vi "WildBugChilGru.vi"() -> ()   [LabVIEW 2014]
uses:
  <vilib>/Utility/miscctls.llb/LVPointTypeDef.ctl
  <vilib>/Utility/xml.llb/Write to XML File(string).vi
  <vilib>/Platform/browser.llb/Open URL in Default Browser (string).vi
  <vilib>/Instr/_visa.llb/VISA Configure Serial Port (Instr).vi
  <vilib>/Analysis/3filter.llb/IIR Filter (DBL).vi
  <vilib>/gmath/NI_Gmath.lvlib
  <vilib>/Analysis/NI_AALBase.lvlib
  <vilib>/ptbypt/NI_PtbyPt.lvlib
panel:
  in  "Grossbild schließen":bool=TRUE
  out "Fahrzeugdaten_gross":string="Fahrzeugdaten"
  out "(c)_gross":string="\n  (c) WildBugGruChil, germanscooterforum.de"
  out "nM_gross":string="\n    4235 1/min"
  out "M_gross":string="15,4 Nm"
  out "Titel_gross":string="Titel"
  out "PS_gross":string="37,6 PS"
  out "nPS_gross":string="\n  6575 1/min"
  out "Y-Koord. Graph-Reset-Button (782)":i32=782
  out "Höhe Leistungs-Graph (646)":u32=646
  in  "FahrzeugdatenZeichenzahl":u8 max=100
  out "Strecke [m]":dbl
  out "dT":dbl=3003.0
  out "Cyclecounter":dbl=3003.0
  out "Datum+Zeit":string="01.12.2021 09:48"
  out "n(Pmax)":dbl=5307.692307692308
  out "Pmax":dbl=17.77254327549455
  out "Lauf abgebrochen":bool
  out "Auto-Datei":string
  out "Auto-Gespeichert":bool
  in  "Auto-Pfad":path
  in  "Auto-Speichern":bool
  out "n(Rolle) [1/min]":dbl=3003.0
  in  "Fahrzeugdaten":string
  out "Ergebnis":string
  out "Pmax":string
  in  "Drucken":bool
  in  "Speichern":bool
  in  "Start":bool
  in  "Ende":bool
  in  "Spenden":bool
  in  "Registerkarte":T1(tab)=enum."Betriebsmodus & Recalc"
  in  "Zündung [Imp/U]":dbl=1.0 format="%#.2f"
  in  "Übersetzung ermitteln aus":T2(ring)
  in  "Getriebe [1:]":dbl=4.0 min=0.0001
  in  "Reifenumfang [m]":dbl=1.222 min=0.0001
  in  "Dauer [s]":u8=5
  in  "nKuWe/nRolle":dbl=0.8 format="%#.3f"
  in  "Lufttemperatur [°C]":dbl=23.2 format="%#.1g"
  in  "Luftdruck [mbar]":dbl=100.34 min=0.0001
  in  "Messung Klimadaten":bool=TRUE
  in  "Filter Zündsignal":bool
  in  "v vom Gas [km/h]":u16=40
  in  "Gleitender Mittelwert":u8=35
  in  "Differenzenquotient":u8=12
  in  "n vom Gas [1/min]":u16=5000
  in  "Verlustmoment M1 [Nm] bei n1":dbl min=0.0
  in  "Rollendrehzahl n1 [1/min]":u16=1 min=1
  in  "Verlustmoment M0 [Nm] bei n = 0":dbl min=0.0
  in  "Rollengeber [Inkr/U]":u16=20 min=1
  in  "Rollenumfang [m]":dbl=0.5 min=0.0001
  in  "Rollenträgheit [kgm²]":dbl=2.0 min=0.0001
  in  "Rollendrehzahl aufzeichnen":bool
  in  "Überschrift Leistungsdiagramm":string
  in  "Recalc":bool
  in  "Leistung":bool=TRUE caption="Messung Klimadaten"
  in  "AFR, EGT":bool caption="Messung Klimadaten"
  in  "Lambda":bool caption="Messung Klimadaten"
  in  "Grossbild":bool
  out "Datenspeicher":T3={"Fahrzeugdaten"="§$", "Auto-Pfad"="01.12.2021 09:48|", "Rolle [Inkr/U]"=20, "Rollenumfang [m]"=0.5, "Rollenträgheit [kgm²]"=2.0, "Zündung [Imp/U]"=1.0, "Getriebe [1:]"=4.0, "Reifenumfang [m] "=1.222, "Grossanzeige"=0.0, "Gl. Mittelwert"=35, "Differenzenquotient"=12, "AFR,EGT"=0, "dT [s]"=0.02, "Strecke [m]"=405.045585106383, "Lufttemperatur [°C]"=23.2, "Mv: n1 [1/min]"=1.0, "Luftdruck [mbar]"=100.34, "nRolle"=array[575 elements], "nWelle"=array[575 elements], "AFR"=array[575 elements], "EGT"=array[575 elements], "Übersetzung ermitteln aus"=0, "[s]"=5.0, "Mv: M0 [Nm]"=0.0, "Mv: M1 [Nm]"=0.0, "n vom Gas [1/min]"=5000.0, "dT-Array [s]"=array[575 elements], [], "Boolesch"=TRUE, "Serielle Schnittstelle"="COM4", "nKuWe/nRolle"=0.8, "v vom Gas [km/h]"=40.0}
  out "COM-Fehlerrate":string="0 / 0,0%"
  in  "Konfiguration:":bool
  out "Füllstand Lesepuffer":u64(slide)=1 scale=1.0..100.0
  out "Lesepuffer":string="\n"
  in  "Serielle Schnittstelle":refnum<visa-resource-name>="COM4"
  in  "Registerkarte 2":enum32{"Seite 1", "Seite 2"}(tab)
  out "Hinterrad\n[km/h]":dbl(knob) scale=0.0..200.0
  out "Welle\n[1/min]":cluster{dbl, dbl}(knob) scale=0.0..14000.0
  out "[°C]":dbl(knob) scale=0.0..800.0 scale format="%#.6g"
  out "AFR":dbl(knob) min=10.0 max=20.0 scale=10.0..20.0
  out "Text Rolle":string="Rolle"
  out "Text Zündung":string="Zündung"
  in  "Reset Skalierung":bool
  out "Untersetzung\nermittelt":bool
  out "Leistungs-Graph":cluster{dbl[], dbl[]}[](graph)
  out "Untersetzung":dbl format="%#.3f"
  out "Untersetzung-Graph":dbl(graph)=1.6366612111292962 caption="Untersetzung"
  out "AFR,EGT-Graph":cluster{dbl[], dbl[]}[](graph)
  # "Leistungsmessung:\n1. Drehzahl konstant halten\n2. START [F1]\n3. Drehzahl weiter halten\n4. bei GO: Vollgas\n5. vom Gas gehen"
  # "WildBugGruChil Dyno v3.2.1"
  # "Untersetzung aus:"
  # "Eingabe <> Messen"
  # "Tacho <> Leistung"
  # "AFR / l &  EGT"
  # "AFR <> l"
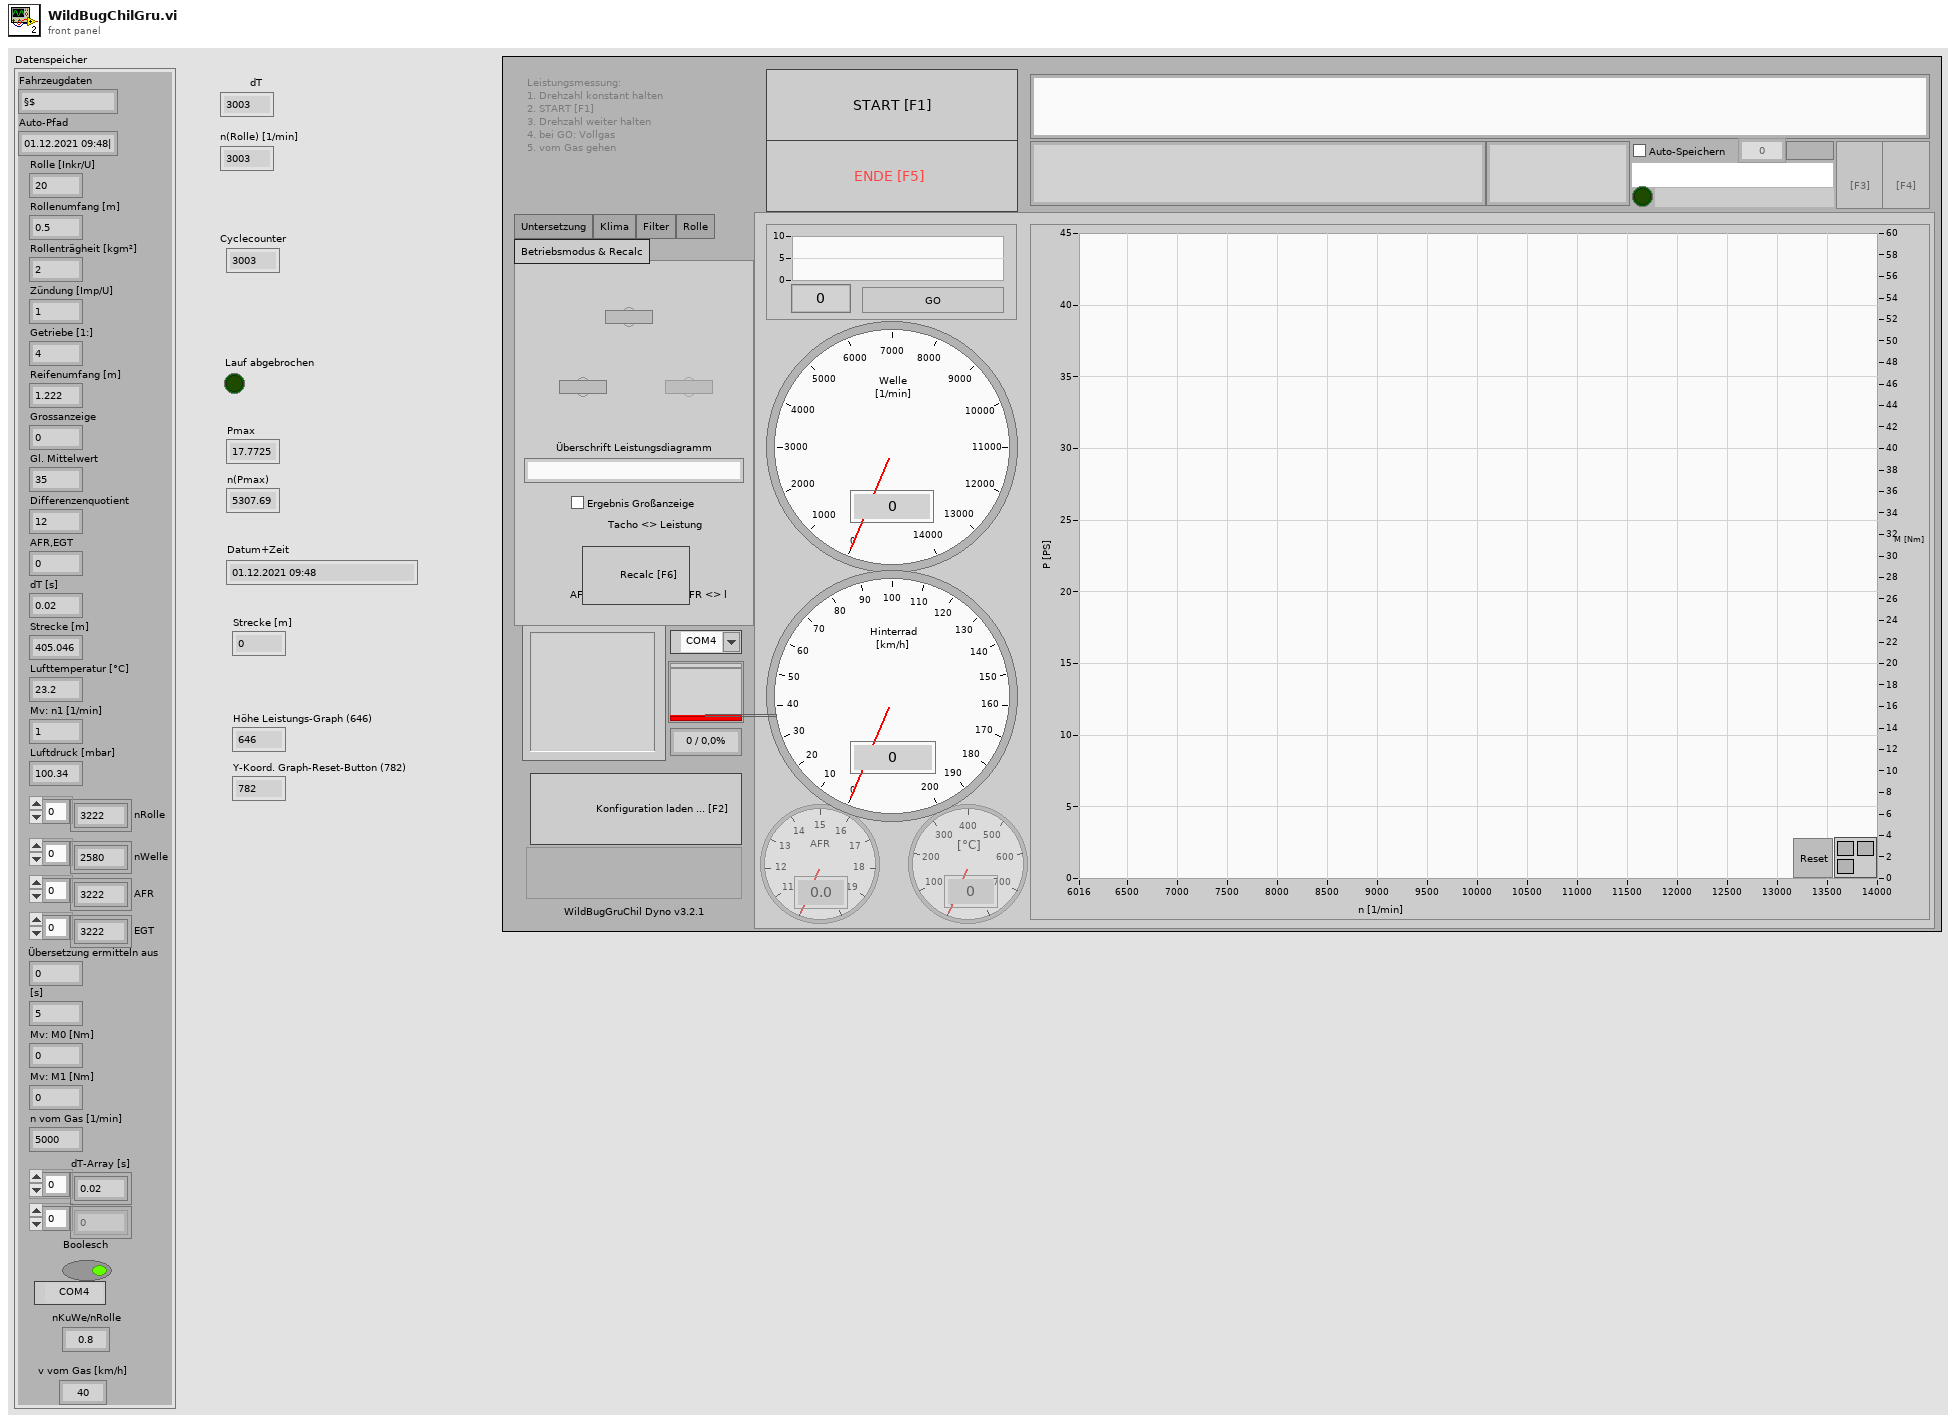
[diagram p1: front panel]
types:
  T1 = enum32{"Untersetzung", "Klima", "Filter", "Rolle", "Betriebsmodus & Recalc"}
  T2 = enum8{"Zündsignal", "Getriebe & Reifen", "nKuWe / nRolle", "Vario (km/h)"}
  T3 = cluster{"Fahrzeugdaten":string, "Auto-Pfad":string, "Rolle [Inkr/U]":u16, "Rollenumfang [m]":dbl, "Rollenträgheit [kgm²]":dbl, "Zündung [Imp/U]":dbl, "Getriebe [1:]":dbl, "Reifenumfang [m] ":dbl, "Grossanzeige":dbl, "Gl. Mittelwert":u8, "Differenzenquotient":u8, "AFR,EGT":u8, "dT [s]":dbl, "Strecke [m]":dbl, "Lufttemperatur [°C]":dbl, "Mv: n1 [1/min]":dbl, "Luftdruck [mbar]":dbl, "nRolle":dbl[], "nWelle":dbl[], "AFR":dbl[], "EGT":dbl[], "Übersetzung ermitteln aus":u8, "[s]":dbl, "Mv: M0 [Nm]":dbl, "Mv: M1 [Nm]":dbl, "n vom Gas [1/min]":dbl, "dT-Array [s]":dbl[], i32[], "Boolesch":bool, "Serielle Schnittstelle":refnum<visa-resource-name>, "nKuWe/nRolle":dbl, "v vom Gas [km/h]":dbl}
  T4 = enum8{"Enabled", "Disabled", "Disabled and Grayed Out"}
  T5 = cluster{string, string, "Rollengeber [Inkr/U]":u16, "Rollenumfang [m]":dbl, "Rollenträgheit [kgm²]":dbl, "Zündung [Imp/U]":dbl, "Getriebe [1:]":dbl, "Reifenumfang [m] ":dbl, dbl, "Gleitender Mittelwert":u8, "Differenzenquotient":u8, u32, dbl, "Strecke [m]":dbl, "Lufttemperatur [°C]":dbl, "Rollendrehzahl n1 [1/min]":u16, "Luftdruck [mbar]":dbl, dbl[], dbl[], dbl[], dbl[], "Übersetzung ermitteln aus":enum8{"Zündsignal", "Getriebe & Reifen", "nKuWe / nRolle", "Vario (km/h)"}, "Dauer [s]":u8, "Verlustmoment M0 [Nm] bei n = 0 ":dbl, "Verlustmoment M1 [Nm] bei n1":dbl, "n vom Gas [1/min]":u16, dbl[], i32[], "Messung Klimadaten":bool, "VISA-Referenz (Ausgang)":refnum<visa-resource-name>, "nKuWe/nRolle":dbl, "v vom Gas [km/h]":u16}
  T6 = typedef "LVPointTypeDef.ctl" = cluster{"Horizontal":i16, "Vertical":i16}
  T7 = enum32{"invalid app kind", "Development System", "Run Time System", "Student Edition", "Embedded LabVIEW", "Evaluation", "Custom"}
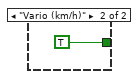
[diagram p3: hidden frame]
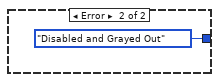
[diagram p5: hidden frame]
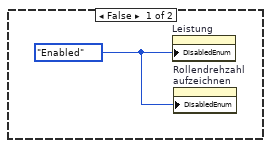
[diagram p6: hidden frame]
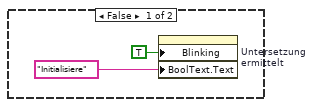
[diagram p7: hidden frame]
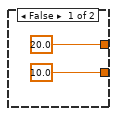
[diagram p8: hidden frame]
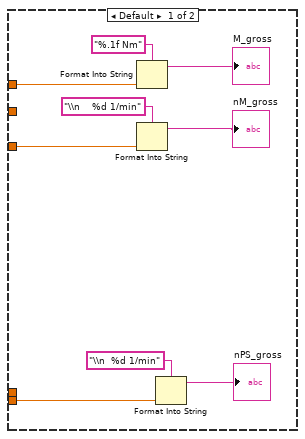
[diagram p11: hidden frame]
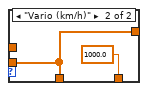
[diagram p18: hidden frame]
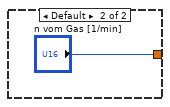
[diagram p19: hidden frame]
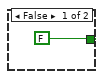
[diagram p20: hidden frame]
diagram:
  w1 = FALSE
  w4 = FALSE
  n1 = while {
    stop <- w14 stop-if-true
    n2 = Wait (ms)(milliseconds to wait=10) -> ()  [unwired: 1 out]
    n3 = local read "Rollendrehzahl aufzeichnen"() -> (w11:bool)
    n4 = local read "Start"() -> (w15:bool)
    n5 = Not(x=w11) -> (.not. x?=w10:bool)
    n6 = And(x="Leistung", y=w10) -> (x .and. y?=w8:bool)
    n7 = Not(x=w8) -> (.not. x?=w12:bool)
    n8 = Boolean To (0,1)(Boolean=w12) -> (0, 1=w13:i16)
    n9 = property on="Registerkarte 2" class="RKElem (strikt)"("Value"=w13) -> ()  [unwired: 2 in, 2 out]
    n10 = case shown="True" w15 {
      tunnel: w8 -> [_ w47]
      frame False {
        w16 = T4."Enabled" ("Deaktiviert")
        n11 = property on="Leistung" class="Bool. (strikt)"("DisabledEnum"=w16) -> ()  [unwired: 2 in, 2 out]
        n12 = property on="Rollendrehzahl aufzeichnen" class="Bool. (strikt)"("DisabledEnum"=w16) -> ()  [unwired: 2 in, 2 out]
      }
      frame True {
        w28 = 0
        w29 = 0.0
        w31 = 0
        w34 = FALSE
        n13 = flat-sequence {
          tunnel: [w89] -> w78
          tunnel: [w88] -> w77
          tunnel: [w86] -> w76
          tunnel: w47 -> [w84]
          tunnel: w78 -> [w106]
          tunnel: w77 -> [w108]
          tunnel: [w101] -> w75
          tunnel: [w106] -> w74
          tunnel: [w108] -> w73
          tunnel: w76 -> [w107]
          tunnel: [w107] -> w72
          tunnel: [w122] -> w71
          tunnel: [w121] -> w46
          tunnel: [w120] -> w45
          tunnel: w75 -> [w122]
          tunnel: w74 -> [w118]
          tunnel: w73 -> [w117]
          tunnel: w72 -> [w119]
          tunnel: w71 -> [w132]
          tunnel: [w132] -> w70
          tunnel: [w131] -> w69
          tunnel: [w130] -> w68
          tunnel: [w128] -> w67
          tunnel: w46 -> [w131]
          tunnel: w45 -> [w130]
          tunnel: [w124] -> w23
          tunnel: [w123] -> w22
          tunnel: ["Gleitender Mittelwert"] -> w56
          tunnel: [w148] -> w57
          tunnel: [w147] -> w58
          tunnel: [w166] -> w59
          tunnel: [w160] -> w54
          tunnel: [w159] -> w55
          tunnel: [w167] -> w60
          tunnel: w70 -> [w167]
          tunnel: w69 -> [w162]
          tunnel: w68 -> [w161]
          tunnel: w67 -> [w166]
          tunnel: [w153] -> w44
          tunnel: [w154] -> w43
          tunnel: [w145] -> w40
          tunnel: w23 -> [w143]
          tunnel: w22 -> [w142]
          frame #0 {
            w94 = u16 0 items=["None", "XON/XOFF", "RTS/CTS", "XON/XOFF & RTS/CTS", "DTR/DSR", "XON/XOFF & DTR/DSR"] ("flow control (0:none)")
            w95 = u16 10 items=["1.0"=10, "1.5"=15, "2.0"=20] ("stop bits (10: 1 bit)")
            w87 = FALSE  # Enable Termination Char (T)
            w90 = u32 10000  # timeout (10sec)
            n14 = And(x="Messung Klimadaten", y=w84) -> (x .and. y?=w86:bool)
            n15 = call-poly "VISA Configure Serial Port"("VISA resource name"="Serielle Schnittstelle", "timeout (10sec)"=w90, "Enable Termination\nChar (T)"=w87, "baud rate (9600)"=u32 115200 ("baudrate (250000)"), "data bits (8)"=u16 8, "parity (0:none)"=enum16{"None", "Odd", "Even", "Mark", "Space"}."None", "stop bits (10: 1 bit)"=w95, "flow control (0:none)"=w94) -> ("VISA resource name out"=w92:refnum<visa-resource-name>, "error out"=w91:errorcluster)  [unwired: 6 in]
            n16 = VISA Clear(VISA resource name=w92, error in (no error)=w91) -> (VISA resource name out=w89:refnum<visa-resource-name>, error out=w88:errorcluster)
          }
          frame #1 {
            w100 = FALSE
            w102 = T4."Disabled and Grayed Out" ("Deaktiviert")
            w109 = 0.0  # Graphen löschen
            w101 = ""
            n17 = case shown="True" w107 {
              frame False {
                n18 = property on="Untersetzung\nermittelt" class="Bool. (strikt)"("Blinking"=TRUE ("Blinkend"), "BoolText.Text"="Initialisiere" ("Beschriftung.Text")) -> ()  [unwired: 2 in, 2 out]
              }
              frame True {
                n19 = Wait (ms)(milliseconds to wait=u32 2000 ("Zu wartende ms")) -> ()  [unwired: 1 out]
                n20 = property on="Untersetzung\nermittelt" class="Bool. (strikt)"("Blinking"=TRUE ("Blinkend"), "BoolText.Text"="Lese Klimadaten" ("Beschriftung.Text")) -> ()  [unwired: 2 in, 2 out]
              }
            }
            n21 = Build Array(w109) -> (w103:dbl[])
            n22 = property on="Auto-Gespeichert" class="Bool. (strikt)"("Value"=w100) -> ()  [unwired: 2 in, 2 out]
            n23 = property on="Lauf abgebrochen" class="Bool. (strikt)"("Value"=w100) -> ()  [unwired: 2 in, 2 out]
            n24 = property on="Untersetzung-Graph" class="SVDiagr (strikt)"("History Data"=w103) -> ()  [unwired: 2 in, 2 out]
            n25 = property on="Drucken" class="Bool. (strikt)"("DisabledEnum"=w102) -> ()  [unwired: 2 in, 2 out]
            n26 = property on="Übersetzung ermitteln aus" class="Enum (strikt)"("DisabledEnum"=w102) -> ()  [unwired: 2 in, 2 out]
            n27 = property on="Konfiguration:" class="Bool. (strikt)"("DisabledEnum"=w102) -> ()  [unwired: 2 in, 2 out]
            n28 = property on="Ende" class="Bool. (strikt)"("DisabledEnum"=w102) -> ()  [unwired: 2 in, 2 out]
            n29 = property on="Leistung" class="Bool. (strikt)"("DisabledEnum"=w102) -> ()  [unwired: 2 in, 2 out]
            n30 = property on="Speichern" class="Bool. (strikt)"("DisabledEnum"=w102) -> ()  [unwired: 2 in, 2 out]
            n31 = property on="Rollendrehzahl aufzeichnen" class="Bool. (strikt)"("DisabledEnum"=w102) -> ()  [unwired: 2 in, 2 out]
            n32 = local write "Pmax"(w101) -> ()
            n33 = local write "COM-Fehlerrate"(w101) -> ()
            n34 = local write "Ergebnis"(w101) -> ()
            n35 = Bundle(w103, w103) -> (w105:cluster{dbl[], dbl[]})  [unwired: 1 in]
            n36 = Bundle(w103, w103) -> (w104:cluster{dbl[], dbl[]})  [unwired: 1 in]
            n37 = Build Array(w105, w104) -> (→"AFR,EGT-Graph" →"Leistungs-Graph":cluster{dbl[], dbl[]}[])
            n38 = local write "Auto-Datei"(w101) -> ()
          }
          frame #2 {
            n39 = control-ref of="Lufttemperatur [°C]"() -> (w115:refnum<vi>)
            n40 = control-ref of="Luftdruck [mbar]"() -> (w116:refnum<vi>)
            n41 = call "MessungKlimadaten(SubVI).vi"("Boolesch"=w119, "Fehler (Eingang, kein Fehler)"=w117, "VISA resource name out"=w118, "Lufttemperatur [°C] (Eingang)"=w115, "Luftdruck [mbar] (Eingang)"=w116) -> ("Fehler (Ausgang)"=w120:errorcluster, "VISA-Referenz (Ausgang)"=w121:refnum<visa-resource-name>)  [unwired: 5 in]
          }
          frame #3 {
            n42 = local read "Lambda"() -> (w125:bool)
            n43 = Wait (ms)(milliseconds to wait=u32 2000 ("Zu wartende ms")) -> ()  [unwired: 1 out]
            n44 = case shown="True" w125 {
              tunnel: [20.0 1.6] -> w123
              tunnel: [10.0 0.4] -> w124
              frame False {
              }
              frame True {
              }
            }
            n45 = call "KorrekturfaktorDin70020 (SubVI).vi"("Lufttemperatur [°C]"="Lufttemperatur [°C]", "Luftdruck [mbar]"="Luftdruck [mbar]") -> ("Korrekturfaktor"=w128:dbl)  [unwired: 9 in]
          }
          frame #4 {
            w141 = 1
            w138 = 0
            w137 = TRUE ("Kontinuierliche Aktualisierung")
            n46 = Concatenate Strings("m" ("String"), "\n") -> (w165:string)
            n47 = property on="AFR,EGT-Graph" class="XYGraph (strikt)"("ActYScl"=w138, "YScale.ScaleFit"=w138, "YScale.Maximum"=w142, "YScale.Minimum"=w143, "ActYScl"=w141, "YScale.ScaleFit"=w138, "YScale.Maximum"=800.0, "YScale.Minimum"=0.0, "XScale.ScaleFit"=w138, "Smooth Update"=w137) -> ()  [unwired: 2 in, 2 out]
            n48 = VISA Write(VISA resource name=w162, write buffer=w165, error in (no error)=w161) -> (VISA resource name out=w159:refnum<visa-resource-name>, error out=w160:errorcluster)  [unwired: 1 out]
            n49 = property on="Leistungs-Graph" class="XYGraph (strikt)"("ActYScl"=w138, "YScale.ScaleFit"=w138, "ActYScl"=w141, "YScale.ScaleFit"=w138, "XScale.ScaleFit"=w138, "Smooth Update"=w137, "Active Plot"=w138, "Plot.Line Width"=2, "Active Plot"=w141, "Plot.Line Width"=w141) -> ()  [unwired: 2 in, 2 out]
            n50 = Divide(x="Gleitender Mittelwert", y=2) -> (x/y=w152:dbl)
            n51 = Round Toward -Infinity(1:w152) -> (0:w145:dbl)
            n52 = local read "Differenzenquotient"() -> (w157:u8)
            n53 = property on="Untersetzung\nermittelt" class="Bool. (strikt)"("Blinking"=FALSE ("Blinkend")) -> ()  [unwired: 2 in, 2 out]
            n54 = call <vilib>:"Smoothing Filter Coefficients.vi"("shape"=1, "half-width"=w145, "type"=0) -> ("forward coefficients"=w148:dbl[], "reverse coefficients"=w147:dbl[])  [unwired: 6 in, 1 out]
            n55 = call <vilib>:"Smoothing Filter Coefficients.vi"("shape"=0, "half-width"=w157, "type"=0) -> ("forward coefficients"=w154:dbl[], "reverse coefficients"=w153:dbl[])  [unwired: 6 in, 1 out]
          }
        }
        n56 = Initialize Array(0.0 ("y"), 0) -> (w24:dbl[])
        n57 = Initialize Array(w28, w28) -> (w27:i32[])
        n58 = while {
          tunnel: w55 -> [w426]
          tunnel: w54 -> [w425]
          shift-right: [w470] -> _
          shift-left: w60 -> [w432]
          shift-right: [w383] -> _
          shift-left: w29 -> [w469]
          shift-right: [w465] -> _
          shift-left: w29 -> [w468]
          shift-right: [w435] -> _
          shift-left: w29 -> [w467]
          shift-right: [w399] -> _
          shift-left: w31 -> [w466]
          shift-right: [w439] -> w63
          shift-left: w29 -> [w420]
          shift-right: [w416] -> w17
          shift-left: w29 -> [w380]
          shift-right: [w436] -> _
          shift-left: w24 -> [w462]
          shift-right: [w419] -> _
          shift-left: w34 -> [w415]
          shift-right: [w459] -> w62
          shift-left: w24 -> [w457]
          shift-right: [w458] -> _
          shift-left: w24 -> [w372]
          shift-right: [w411] -> w36
          shift-left: w24 -> [w456]
          shift-right: [w453] -> _
          shift-left: w24 -> [w454]
          shift-right: [w452] -> w48
          shift-left: w24 -> [w455]
          shift-right: [w410] -> w37
          shift-left: w24 -> [w374]
          shift-right: [w409] -> w38
          shift-left: w24 -> [w375]
          tunnel: [w451] -> w66
          shift-right: [w447] -> w65
          shift-left: w31 -> [w449]
          tunnel: [w450] -> w51
          tunnel: [w414] -> w64
          tunnel: ["Rollenumfang [m]"] -> w26
          shift-right: [w446] -> _
          shift-left: w34 -> [w424]
          shift-right: [w440] -> _
          shift-left: -5 -> [w445]
          shift-right: [w441] -> _
          shift-left: w29 -> [w444]
          shift-right: [w442] -> _
          shift-left: w29 -> [w443]
          shift-right: [w423] -> w25
          shift-left: w24 -> [w438]
          shift-right: [w369] -> _
          shift-left: _ -> [w434]
          shift-right: [w437] -> w61
          shift-left: w27 -> [w433]
          tunnel: [w431] -> w52
          tunnel: w59 -> [w385]
          tunnel: w58 -> [w427]
          tunnel: w57 -> [w408]
          tunnel: w56 -> [w384]
          tunnel: w44 -> [w422]
          tunnel: w43 -> [w421]
          shift-right: [w401] -> w41
          shift-left: w24 -> [w403]
          shift-right: [w400] -> w35
          shift-left: w24 -> [w373]
          tunnel: w40 -> [w392]
          tunnel: [w385] -> w39
          shift-right: [w367] -> _
          shift-left: _ -> [w363]
          shift-right: [w366] -> _
          shift-left: _ -> [w362]
          shift-right: [w360] -> w20
          shift-left: w24 -> [w365]
          shift-right: [w359] -> w21
          shift-left: w24 -> [w364]
          i -> [w405]
          stop <- w451 stop-if-true
          w398 = 3  # Vario(km/h)
          n59 = property class="Instr"(reference=w426, error in=w425) -> (reference out=w430:refnum<visa-resource-name>, error out=w429:errorcluster, "Serial Settings:Number of Bytes at Serial Port"=w388:u32)
          n60 = Greater?(x=w388, y=u32 1 ("min. Bytes")) -> (0:w389:bool)
          n61 = control-ref of="Füllstand Lesepuffer"() -> (w413:refnum<vi>)
          n62 = Select(t=w388, s=w389, f=u32 0 ("Bytes at Port")) -> (s? t:f=w387:u32)
          n63 = local read "AFR, EGT"() -> (w358:bool)
          n64 = call "Stringhandling(SubVI)0.0.2.vi"("Slide (Eingang)"=w413, "Numerisch (Eingang)"=w466, "VISA-Referenz (Eingang)"=w430, "MessFrequenz [Hz]"=w467, "Bytes at Port"=w387, "Fehler (Eingang, kein Fehler)"=w429, "Cyclecounter (Eingang)"=w434, "Rolle[Hz]"=w468, "Temp[°C] (Eingang)"=w362, "AFR (Eingang)"=w363, "String (Eingang)"=w432, "Zündung [Hz] (Eingang)"=w469, "AFR+EGT"=w358) -> ("Lesepuffer"=→"Lesepuffer":string, "Numerisch (Ausgang)"=w399:i32, "String (Ausgang)"=w470:string, "Temp[°C] (Ausgang)"=w366:dbl, "AFR (Ausgang)"=w367:dbl, "VISA-Referenz (Ausgang)"=w431:refnum<visa-resource-name>, "Zündung [Hz] (Ausgang)"=w382:dbl, "Rolle [Hz]"=w465:dbl, "Messfrequenz [Hz]"=w435:dbl, "Cyclecounter (Ausgang)"=w369:i32, "Fehler (Ausgang)"=w450:errorcluster)  [unwired: 4 in]
          "Füllstand Lesepuffer" <- w399
          "Cyclecounter" <- w369
          n65 = case shown="True" "AFR, EGT" {
            tunnel: w363 -> [_ w475]
            tunnel: w366 -> [_ w473]
            tunnel: w362 -> [_ w472]
            tunnel: w367 -> [_ w471]
            frame False {
            }
            frame True {
              n66 = Not Equal?(x=w471, y=w475) -> (x != y?=w476:bool)
              n67 = case shown="True" w476 {
                tunnel: w471 -> [_ w479]
                frame False {
                }
                frame True {
                  n68 = Multiply(x=0.06802721088435375, y=w479) -> (x*y=w481:dbl)
                  n69 = local read "Lambda"() -> (w482:bool)
                  n70 = Select(t=w481, s=w482, f=w479) -> (s? t:f=→"AFR":dbl)
                }
              }
              n71 = Not Equal?(x=w473, y=w472) -> (x != y?=w474:bool)
              n72 = case shown="True" w474 {
                tunnel: w473 -> [_ w477]
                frame False {
                }
                frame True {
                  "[°C]" <- w477
                }
              }
            }
          }
          n73 = local read "Übersetzung ermitteln aus"() -> (w397:T2)
          n74 = Not Equal?(x=w398, y=w397) -> (x != y?=w395:bool)
          n75 = And(x="Filter Zündsignal", y=w395) -> (x .and. y?=w393:bool)
          n76 = Select(t=w392, s=w393, f=0) -> (s? t:f=w381:dbl)
          n77 = call <vilib>:"Median Filter PtByPt.vi"("initialize"=TRUE, "rank"=w381, "x"=w382) -> ("Filtered x"=w383:dbl)  [unwired: 1 in, 1 out]
          n78 = Not Equal?(x=w434, y=w369) -> (x != y?=w370:bool)
          n79 = case "Case-Struktur" shown="True" w370 {
            tunnel: w383 -> [w777 w798]
            tunnel: w465 -> [w776 w797]
            tunnel: [w777 w786] -> w464
            tunnel: [w776 w783] -> w463
            tunnel: w435 -> [_ w793]
            tunnel: w420 -> [w775 _]
            tunnel: [w775 w781] -> w439
            tunnel: w380 -> [_ w784]
            tunnel: "Rollenumfang [m]" -> [_ w796]
            tunnel: w397 -> [_ w790]
            frame False {
            }
            frame True {
              w801 = 60.0 ("y")
              n80 = Reciprocal "Abtastzeit [s]"(x=w793) -> (1/x=w781:dbl)
              "dT" <- w781
              n81 = Divide "R [1/s]"(x=w797, y="Rollengeber [Inkr/U]") -> (x/y=w785:dbl)
              n82 = Divide(x=w798, y="Zündung [Imp/U]") -> (x/y=w800:dbl)
              n83 = Multiply "[m/s]"(x=w785, y=w796) -> (x*y=w782:dbl)
              n84 = Multiply(x=w782, y=w781) -> (x*y=w778:dbl)
              n85 = Multiply "nZ gemessen [1/min]"(x=w800, y=w801) -> (x*y=w786:dbl)
              n86 = Multiply "nR [1/min]"(x=w801, y=w785) -> (x*y=w783:dbl)
              "n(Rolle) [1/min]" <- w783
              n87 = local read "Strecke [m]"() -> (w779:dbl)
              n88 = Multiply "nZ berechnet [1/min]"(x=w784, y=w783) -> (x*y=w788:dbl)
              n89 = case shown="Standard" w790 {
                tunnel: [w803 w804] -> w789
                tunnel: w788 -> [w803 w805]
                tunnel: [w802 w805] -> w787
                tunnel: w786 -> [w802 w804]
                frame Default {
                }
                frame "Vario (km/h)" {
                }
              }
              n90 = Add(x=w779, y=w778) -> (x+y=→"Strecke [m]":dbl)
              n91 = Bundle(w789, w787) -> (→"Welle\n[1/min]":cluster{dbl, dbl})  [unwired: 1 in]
              n92 = Multiply ("[km/h]")(x=w782, y=3.6) -> (x*y=→"Hinterrad\n[km/h]":dbl)
            }
          }
          n93 = case shown="True" w370 {
            tunnel: w445 -> [w526 w537]
            tunnel: [w526 w549] -> w440
            tunnel: w444 -> [w525 w548]
            tunnel: [w525 w534] -> w441
            tunnel: w443 -> [w524 w547]
            tunnel: [w524 w535] -> w442
            tunnel: w369 -> [_ w533]
            tunnel: w433 -> [w523 w532]
            tunnel: [w523 w536] -> w437
            frame False {
            }
            frame True {
              n94 = Build Array (concatenate)(w532, w533) -> (w536:i32[])
              n95 = Greater Or Equal To 0?(x=w537) -> (x >= 0?=w538:bool)
              n96 = case shown="True" w538 {
                tunnel: [w550 w561] -> w534
                tunnel: [w550 w562] -> w535
                tunnel: [w551 w553] -> w549
                tunnel: w548 -> [_ w555]
                tunnel: w547 -> [_ w563]
                tunnel: w533 -> [w551 w552]
                tunnel: w537 -> [_ w553]
                frame False {
                  w550 = 1.0
                }
                frame True {
                  w559 = 65536.0
                  n97 = Add(x=w553, y=w555) -> (x+y=w554:dbl)
                  n98 = Divide(x=w554, y=w559) -> (x/y=w564:dbl)
                  n99 = Increment(x=w563) -> (x+1=w562:dbl)
                  n100 = Round Toward -Infinity(1:w564) -> (0:w560:dbl)
                  n101 = Multiply(x=w560, y=w559) -> (x*y=w558:dbl)
                  n102 = Add(x=w558, y=w552) -> (x+y=w557:dbl)
                  n103 = Increment(x=w557) -> (x+1=w556:dbl)
                  n104 = Subtract(x=w556, y=w553) -> (x-y=w561:dbl)
                }
              }
              n105 = Subtract(x=w534, y=w535) -> (x-y=w529:dbl)
              n106 = Decrement(x=w529) -> (x-1=w528:dbl)
              n107 = Max & Min(x=0, y=w528) -> (max(x,y)=w527:dbl)  [unwired: 1 out]
              n108 = Divide(x=w527, y=w534) -> (x/y=w541:dbl)
              n109 = Greater Than 0?(x=w527) -> (x > 0?=w531:bool)
              n110 = Select(t=u32 16711680, s=w531, f=u32 0) -> (s? t:f=w542:u32)
              n111 = Multiply(x=w541, y=100.0) -> (x*y=w539:dbl)
              n112 = property on="COM-Fehlerrate" class="Str"("Text.TextColor"=w542) -> ()  [unwired: 2 in, 2 out]
              n113 = Format Into String(format string="%d / %.1f%%" ("Format-String"), w527, w539) -> (resulting string=→"COM-Fehlerrate":string)  [unwired: 2 in, 1 out]
            }
          }
          n114 = case shown="\"Vario (km/h)\"" w397 {
            tunnel: [w515 "n vom Gas [1/min]"] -> w414
            frame "Vario (km/h)" {
              n115 = local read "Rollenumfang [m]"() -> (w516:dbl)
              n116 = Divide(x="v vom Gas [km/h]", y=w516) -> (x/y=w514:dbl)
              n117 = Multiply(x=w514, y=16.66666667) -> (x*y=w515:dbl)
            }
            frame Default {
            }
          }
          n118 = case shown="True" w370 {
            tunnel: w464 -> [_ w625]
            tunnel: w463 -> [_ w678]
            tunnel: "Rollenumfang [m]" -> [_ w679]
            tunnel: [w580 w608] -> w416
            tunnel: w380 -> [w569 w608]
            tunnel: w415 -> [w581 w627]
            tunnel: w462 -> [w582 w682]
            tunnel: [w581 w654] -> w419
            tunnel: [w582 w681] -> w436
            tunnel: w427 -> [_ w624]
            tunnel: w408 -> [_ w623]
            tunnel: [w579 w605] -> w459
            tunnel: [w578 w606] -> w458
            tunnel: w457 -> [w579 w677]
            tunnel: w372 -> [w578 _]
            tunnel: w384 -> [_ w622]
            tunnel: [w577 w612] -> w411
            tunnel: w456 -> [w577 _]
            tunnel: [w576 w635] -> w453
            tunnel: w454 -> [w576 _]
            tunnel: [w575 w619] -> w452
            tunnel: w455 -> [w575 _]
            tunnel: [w574 w613] -> w410
            tunnel: w374 -> [w574 _]
            tunnel: [w573 w671] -> w409
            tunnel: w375 -> [w573 _]
            tunnel: w385 -> [_ w621]
            tunnel: w449 -> [w572 w665]
            tunnel: w414 -> [_ w656]
            tunnel: [w572 w664] -> w447
            tunnel: w424 -> [w571 w661]
            tunnel: [w571 w660] -> w446
            tunnel: w439 -> [_ w659]
            tunnel: [w570 w629] -> w423
            tunnel: w438 -> [w570 w658]
            tunnel: w422 -> [_ w642]
            tunnel: w421 -> [_ w641]
            tunnel: w403 -> [w568 w626]
            tunnel: [w568 w607] -> w401
            tunnel: [w567 w603] -> w400
            tunnel: w373 -> [w567 _]
            tunnel: w392 -> [_ w604]
            tunnel: w367 -> [_ w602]
            tunnel: w366 -> [_ w601]
            tunnel: w365 -> [w566 w600]
            tunnel: w364 -> [w565 w599]
            tunnel: [w566 w598] -> w360
            tunnel: [w565 w597] -> w359
            frame False {
              n119 = case shown="False" w581 {
                tunnel: w582 -> [w589 _]
                tunnel: [w583 w596] -> w580
                tunnel: w569 -> [_ w596]
                frame False {
                  n120 = local read "Übersetzung ermitteln aus"() -> (w586:T2)
                  n121 = call <vilib>:"Measures of Mean.vi"("percent (trim)"=20.0, "type"=3, "x array"=w589) -> ("mean value"=w584:dbl)  [unwired: 7 in, 1 out]
                  n122 = Equal To 0? "aus Zündsignal?"(x=w586) -> (x = 0?=w585:bool)
                  n123 = case shown="True" w585 {
                    tunnel: w584 -> [w590 w595]
                    tunnel: [w590 w591] -> w583
                    frame False {
                    }
                    frame True {
                      w592 = 1000.0
                      n124 = Multiply(x=w595, y=w592) -> (x*y=w594:dbl)
                      n125 = Round To Nearest(number=w594) -> (nearest integer value=w593:dbl)
                      n126 = Divide(x=w593, y=w592) -> (x/y=w591:dbl)
                    }
                  }
                }
                frame True {
                }
              }
            }
            frame True {
              w668 = 0.00135962  # [W] in [PS]
              w673 = 0.10471975511965978  # 2*Pi/60
              # "Einzelne Ausreisser (Zündsignal) werden\nam besten mit Median-Filter eliminiert"
              n127 = Not(x=w627) -> (.not. x?=w632:bool)
              n128 = local read "Leistung"() -> (w631:bool)
              n129 = Square(x=w608) -> (x^2=w672:dbl)
              n130 = Or(x=w631, y=w632) -> (x .or. y?=w630:bool)
              n131 = case shown="True" w630 {
                tunnel: w678 -> [_ w702]
                tunnel: w677 -> [w686 w701]
                tunnel: w659 -> [_ w700]
                tunnel: w658 -> [w687 w699]
                tunnel: [w686 w698] -> w605
                tunnel: [w687 w697] -> w629
                tunnel: w626 -> [w685 w696]
                tunnel: [w685 w695] -> w607
                tunnel: w625 -> [_ w694]
                tunnel: w602 -> [_ w693]
                tunnel: w601 -> [_ w692]
                tunnel: w600 -> [w684 w691]
                tunnel: w599 -> [w683 w690]
                tunnel: [w684 w689] -> w598
                tunnel: [w683 w688] -> w597
                frame False {
                }
                frame True {
                  n132 = Build Array (concatenate) "AFR in Array einf."(w691, w693) -> (w689:dbl[])
                  n133 = Build Array (concatenate) "EGT in Array einf."(w690, w692) -> (w688:dbl[])
                  n134 = Build Array (concatenate) "nRolle in Array einf."(w701, w702) -> (w698:dbl[])
                  n135 = Build Array (concatenate) "dT in Array einf."(w699, w700) -> (w697:dbl[])
                  n136 = Build Array (concatenate) "nWelle in Array einf."(w696, w694) -> (w695:dbl[])
                }
              }
              n137 = local read "Übersetzung ermitteln aus"() -> (w633:T2)
              n138 = Divide(x="Rollenträgheit [kgm²]", y=w672) -> (x/y=w620:dbl)
              n139 = case shown="\"Getriebe & Reifen\"" w633 {
                tunnel: w625 -> [w767 _ _ _]
                tunnel: w678 -> [w766 _ _ _]
                tunnel: [w765 w771 "nKuWe/nRolle" 1.0] -> w680
                tunnel: w679 -> [_ w772 _ _]
                frame "Zündsignal" {
                  n140 = Divide(x=w767, y=w766) -> (x/y=w765:dbl)
                }
                frame "Getriebe & Reifen" {
                  n141 = Divide(x=w772, y="Reifenumfang [m]") -> (x/y=w770:dbl)
                  n142 = Multiply(x=w770, y="Getriebe [1:]") -> (x*y=w771:dbl)
                }
                frame "nKuWe / nRolle" {
                }
                frame "Vario (km/h)" {
                }
              }
              n143 = Multiply(x=w621, y=w620) -> (x*y=w618:dbl)
              n144 = local read "Differenzenquotient"() -> (w640:u8)
              n145 = Multiply(x=2, y=w640) -> (x*y=w638:i32)
              n146 = Increment(x=w638) -> (x+1=w636:i32)
              n147 = Index Array(array=w605, index=1 ("Index")) -> (element=w652:dbl)
              n148 = Index Array(array=w629, index=1 ("Index")) -> (element=w646:dbl)
              n149 = Initialize Array(w652, w622) -> (w651:dbl[])
              n150 = Initialize Array(w646, w636) -> (w644:dbl[])
              n151 = Insert Into Array(array=w605, index=0 ("Index"), new element=w651) -> (w649:dbl[])
              n152 = Insert Into Array(array=w629, index=0 ("Index"), new element=w644) -> (w643:dbl[])
              n153 = call-poly <vilib>:"IIR Filter.vi"("Forward Coefficients"=w623, "Reverse Coefficients"=w624, "X"=w649) -> ("Filtered X"=w648:dbl[])  [unwired: 1 in, 1 out]
              n154 = call-poly <vilib>:"IIR Filter.vi"("Forward Coefficients"=w641, "Reverse Coefficients"=w642, "X"=w643) -> ("Filtered X"=w637:dbl[])  [unwired: 1 in, 1 out]
              n155 = case shown="False" w627 {
                selector: w627 -> [_ w764]
                tunnel: w680 -> [w752 _]
                tunnel: w682 -> [w754 w763]
                tunnel: [w749 w764] -> w676
                tunnel: [w753 w763] -> w681
                tunnel: w661 -> [w751 w762]
                tunnel: [w749 w762] -> w660
                tunnel: w633 -> [w748 _]
                frame False {
                  n156 = Build Array (concatenate)(w754, w752) -> (w753:dbl[])
                  n157 = case shown="\"Zündsignal\"" w748 {
                    tunnel: ["Dauer [s]" 0.0 ("Dauer [s]")] -> w750
                    frame "Zündsignal" {
                      n158 = property on="Untersetzung\nermittelt" class="Bool. (strikt)"("Blinking"=TRUE ("Blinkend"), "BoolText.Text"="Ermittle Übersetzung" ("Boolescher Text.Text")) -> ()  [unwired: 2 in, 2 out]
                    }
                    frame Default {
                    }
                  }
                  n159 = call "Verstrichene Zeit"("Time Target (s)"=w750, "Reset"=w751) -> ("Time has Elapsed"=w749:bool)  [unwired: 10 in, 7 out]
                  n160 = case shown="True" w749 {
                    frame False {
                    }
                    frame True {
                      n161 = property on="Untersetzung\nermittelt" class="Bool. (strikt)"("Blinking"=FALSE ("Blinkend"), "BoolText.Text"="Go" ("Boolescher Text.Text")) -> ()  [unwired: 2 in, 2 out]
                      n162 = property on="Strecke [m]" class="DigWert (strikt)"("Value"=0.0) -> ()  [unwired: 2 in, 2 out]
                    }
                  }
                  "Untersetzung-Graph" <- w752
                }
                frame True {
                }
              }
              n163 = Array Subset "Rolle gefiltert [1/min]"(array=w648, index=w622) -> (w606:dbl[])  [unwired: 1 in]
              n164 = Array Subset "dT gefiltert [s]"(array=w637, index=w636) -> (w634:dbl[])  [unwired: 1 in]
              n165 = Array Size "Array-Größe"(array=w606) -> (size(s)=w674:i32)
              n166 = Greater?(x=w674, y=w622) -> (0:w675:bool)
              n167 = call <vilib>:"Median Filter.vi"("right rank"=w604, "left rank"=w604, "X"=w607) -> ("Filtered X"=w603:dbl[])  [unwired: 7 in, 1 out]
              n168 = Multiply "* i"(x=w606, y=w608) -> (x*y=w612:dbl[])
              n169 = Multiply(x=w612, y=w673) -> (x*y=w635:dbl[])
              n170 = And(x=w676, y=w675) -> (x .and. y?=w654:bool)
              n171 = Array Size "Array-Größe"(array=w635) -> (size(s)=w628:i32)
              n172 = Decrement(x=w628) -> (x-1=w666:i32)
              n173 = Select(t=w656, s=w654, f=1000000.0) -> (s? t:f=w657:dbl)
              n174 = Initialize Array(0.0 ("y"), 0) -> (w614:dbl[])
              n175 = for {
                N: w628 -> [_]
                tunnel: "Differenzenquotient" -> [w725]
                tunnel: w635 -> [w732]
                tunnel: w666 -> [w724]
                shift-right: [w729] -> w619
                shift-left: w614 -> [w730]
                tunnel: w612 -> [w707] mode=indexing
                tunnel: w665 -> [w717]
                tunnel: w657 -> [w727]
                tunnel: [w718] -> w664
                tunnel: w627 -> [w716]
                tunnel: w634 -> [w713] mode=indexing
                tunnel: "Rollendrehzahl n1 [1/min]" -> [w710]
                tunnel: "Verlustmoment M1 [Nm] bei n1" -> [w709]
                tunnel: "Verlustmoment M0 [Nm] bei n = 0" -> [w708]
                shift-right: [w706] -> w611
                shift-left: w614 -> [w705]
                tunnel: w606 -> [w703] mode=indexing
                i -> [w714]
                stop <- w711 stop-if-true
                # "Beschleunigung a(i) berechnen solange bis n(i) > nSchwelle & a(i) < 0"
                n176 = call "Verlustmoment (SubVI).vi"("n [1/min"=w703, "Verlustmoment M0 [Nm] bei n = 0"=w708, "Verlustmoment M1 [Nm] bei n1"=w709, "Rollendrehzahl n1 [1/min]"=w710) -> ("Mv"=w704:dbl)  [unwired: 7 in]
                n177 = Subtract(x=w724, y=w725) -> (x-y=w726:i32)
                n178 = Multiply(x=w713, y=2.0) -> (x*y=w715:dbl)
                n179 = Subtract(x=w714, y=w725) -> (x-y=w745:i32)
                n180 = Add(x=w714, y=w725) -> (x+y=w739:i32)
                n181 = Greater Or Equal?(x=w714, y=w725) -> (x >= y?=w721:bool)
                n182 = Less Or Equal?(x=w714, y=w726) -> (x <= y?=w722:bool)
                n183 = Greater?(x=w707, y=w727) -> (0:w728:bool)
                n184 = Max & Min(x=w724, y=w739) -> (min(x,y)=w740:i32)  [unwired: 1 out]
                n185 = Max & Min(x=w745, y=0) -> (max(x,y)=w743:i32)  [unwired: 1 out]
                n186 = Subtract(x=w740, y=w714) -> (x-y=w741:i32)
                n187 = Subtract(x=w714, y=w743) -> (x-y=w742:i32)
                n188 = Max & Min(x=w742, y=w741) -> (min(x,y)=w733:i32)  [unwired: 1 out]
                n189 = Add(x=w714, y=w733) -> (x+y=w738:i32)
                n190 = Subtract(x=w714, y=w733) -> (x-y=w737:i32)
                n191 = Multiply(x=w733, y=w715) -> (x*y=w731:dbl)
                n192 = Index Array(array=w732, index=w738) -> (element=w735:dbl)
                n193 = Index Array(array=w732, index=w737) -> (element=w736:dbl)
                n194 = Subtract(x=w735, y=w736) -> (x-y=w734:dbl)
                n195 = Divide(x=w734, y=w731) -> (x/y=w723:dbl)
                n196 = Less Than 0?(x=w723) -> (x < 0?=w720:bool)
                n197 = Less Or Equal To 0?(x=w717) -> (x <= 0?=w719:bool)
                n198 = Build Array (concatenate)(w730, w723) -> (w729:dbl[])
                n199 = Compound Arithmetic op=AND "n(i) > nSchwelle\n& a(i) < 0"(w720, w728, w719, w721, w722, w716) -> (w711:bool)
                n200 = case shown="False" w711 {
                  tunnel: w714 -> [_ w747]
                  tunnel: [w746 w747] -> w718
                  tunnel: w717 -> [w746 _]
                  frame False {
                  }
                  frame True {
                  }
                }
                n201 = Build Array (concatenate) "Mv Rolle"(w705, w704) -> (w706:dbl[])
              }
              n202 = Divide ": i"(x=w611, y=w608) -> (x/y=w610:dbl[])
              n203 = Multiply "* J' * korr"(x=w618, y=w619) -> (x*y=w609:dbl[])
              n204 = Add(x=w609, y=w610) -> (x+y=w613:dbl[])
              n205 = Multiply(x=w635, y=w613) -> (x*y=w667:dbl[])
              n206 = Multiply(x=w668, y=w667) -> (x*y=w671:dbl[])
            }
          }
          "Untersetzung\nermittelt" <- w419
          n207 = local read "Übersetzung ermitteln aus"() -> (w402:T2)
          n208 = Quotient & Remainder(x=w405, y=500) -> (x-y*floor(x/y)=w407:i32)  [unwired: 1 out]
          n209 = Equal To 0? "aus Zündsignal?"(x=w402) -> (x = 0?=w418:bool)
          n210 = Equal To 0?(x=w407) -> (x = 0?=w406:bool)
          n211 = local read "Leistung"() -> (w377:bool)
          n212 = local read "Rollendrehzahl aufzeichnen"() -> (w379:bool)
          n213 = And(x=w419, y=w418) -> (x .and. y?=w417:bool)
          n214 = case shown="True" w406 {
            tunnel: w411 -> [_ w508]
            tunnel: w410 -> [_ w501]
            tunnel: w409 -> [_ w495]
            tunnel: w402 -> [_ w502]
            tunnel: "Rollenumfang [m]" -> [_ w507]
            tunnel: w400 -> [_ w500]
            tunnel: w360 -> [_ w487]
            tunnel: w359 -> [_ w485]
            frame False {
            }
            frame True {
              w488 = 0.06802721088435375  # AFR --> Lambda
              # "Livegraph"
              # "Skal-Y2"
              # "Skal-Y1"
              # "Skal-X"
              n215 = control-ref of="Leistungs-Graph"() -> (w496:refnum<vi>)
              n216 = call "n2v (SubVI).vi"("Übersetzung ermitteln aus"=w502, "Array (Eingang)"=w508, "Rollenumfang [m]"=w507) -> ("Array (Ausgang)"=w486:dbl[])  [unwired: 7 in, 1 out]
              n217 = case shown="Standard" w502 {
                tunnel: [w510 w512] -> w494
                tunnel: w501 -> [w510 _]
                tunnel: w500 -> [_ w512]
                tunnel: [w510 w512] -> w499
                tunnel: [10.0 1000.0] -> w497
                frame Default {
                }
                frame "Vario (km/h)" {
                }
              }
              n218 = call "Scale_Graph_Y (SubVI).vi"("AktYSkl"=1, "Divisor"=w497, "Array"=w499, "Faktor"=2.5, "XYGraph (Eingang)"=w496) -> ()  [unwired: 7 in]
              n219 = local read "Lambda"() -> (w484:bool)
              n220 = call "Scale_Graph_Y (SubVI).vi"("AktYSkl"=0, "Divisor"=10.0, "Array"=w495, "Faktor"=1.0, "XYGraph (Eingang)"=w496) -> ()  [unwired: 7 in]
              n221 = call "Scale_Graph_X (SubVI).vi"("Array"=w486, "Übersetzung ermitteln aus"=w502, "XYGraph (Eingang)"=w496) -> ("xMax (Ausgang)"=w492:dbl, "xMin (Ausgang)"=w493:dbl)  [unwired: 7 in]
              n222 = control-ref of="AFR,EGT-Graph"() -> (w489:refnum<vi>)
              n223 = Multiply(x=w488, y=w487) -> (x*y=w490:dbl[])
              n224 = property on="AFR,EGT-Graph" class="XYGraph (strikt)"("XScale.Minimum"=w493, "XScale.Maximum"=w492) -> ()  [unwired: 2 in, 2 out]
              n225 = Select(t=w490, s=w484, f=w487) -> (s? t:f=w491:dbl[])
              n226 = call "UpdateGraph (SubVI).vi"("x"=w486, "Y2"=w485, "Y1"=w491, "XYGraph (Eingang)"=w489) -> ()  [unwired: 8 in]
              n227 = call "UpdateGraph (SubVI).vi"("x"=w486, "Y2"=w494, "Y1"=w495, "XYGraph (Eingang)"=w496) -> ()  [unwired: 8 in]
            }
          }
          n228 = Select(t=w416, s=w419, f=0.0) -> (s? t:f=→"Untersetzung":dbl)
          n229 = case shown="True" w417 {
            tunnel: w416 -> [_ w522]
            frame False {
            }
            frame True {
              n230 = local write "nKuWe/nRolle"(w522) -> ()
            }
          }
          n231 = Not(x=w379) -> (.not. x?=w378:bool)
          n232 = And(x=w377, y=w378) -> (x .and. y?=w376:bool)
          n233 = case shown="True" w376 {
            tunnel: [FALSE w521] -> w448
            tunnel: w447 -> [_ w520]
            frame False {
            }
            frame True {
              n234 = Greater Than 0?(x=w520) -> (x > 0?=w521:bool)
            }
          }
          n235 = local read "Start"() -> (w428:bool)
          n236 = Not(x=w428) -> (.not. x?=w371:bool)
          n237 = case shown="True" w371 {
            frame False {
            }
            frame True {
              n238 = property on="Lauf abgebrochen" class="Bool. (strikt)"("Value"=TRUE) -> ()  [unwired: 2 in, 2 out]
            }
          }
          n239 = Or(x=w448, y=w371) -> (x .or. y?=w451:bool)
        }
        n240 = VISA Clear(VISA resource name=w52, error in (no error)=w51) -> (VISA resource name out=w49:refnum<visa-resource-name>, error out=w53:errorcluster)
        n241 = VISA Close(VISA resource name=w49, error in (no error)=w53) -> ()  [unwired: 1 out]
        n242 = case shown="True" w66 {
          tunnel: w36 -> [_ w261]
          tunnel: w37 -> [_ w262]
          tunnel: w38 -> [_ w263]
          tunnel: w65 -> [_ w252]
          tunnel: w48 -> [_ w293]
          tunnel: w64 -> [_ w292]
          tunnel: w26 -> [_ w276]
          tunnel: w39 -> [_ w271]
          tunnel: w17 -> [_ w233]
          tunnel: w35 -> [_ w260]
          tunnel: w21 -> [_ w250]
          tunnel: w20 -> [_ w249]
          frame False {
          }
          frame True {
            w277 = 0.06
            n243 = Array Subset "P"(array=w263, length=w252) -> (w267:dbl[])  [unwired: 1 in]
            n244 = Array Subset "n"(array=w261, length=w252) -> (w265:dbl[])  [unwired: 1 in]
            n245 = Array Subset "M"(array=w262, length=w252) -> (w266:dbl[])  [unwired: 1 in]
            n246 = Array Subset "alpha"(array=w293, length=w252) -> (w294:dbl[])  [unwired: 1 in]
            n247 = Array Subset "nWelle"(array=w260, length=w252) -> (w264:dbl[])  [unwired: 1 in]
            n248 = Array Subset "AFR"(array=w249, length=w252) -> (w254:dbl[])  [unwired: 1 in]
            n249 = Array Subset "EGT"(array=w250, length=w252) -> (w253:dbl[])  [unwired: 1 in]
            n250 = property on="Ergebnis" class="Str"("Text.FontSize"=18) -> ()  [unwired: 2 in, 2 out]
            n251 = Array Size(array=w294) -> (size(s)=w295:i32)
            n252 = for {
              N: w295 -> [w357]
              tunnel: w293 -> [w354]
              tunnel: w261 -> [w351]
              tunnel: w292 -> [w348]
              tunnel: [w346] -> w285
              i -> [w352]
              stop <- w347 stop-if-true
              # "Beginn mit n(i)<nSchwelle &  a(i)<0 wegschneiden"
              n253 = Decrement(x=w357) -> (x-1=w356:i32)
              n254 = Subtract(x=w356, y=w352) -> (x-y=w346:i32)
              n255 = Index Array(array=w351, index=w346) -> (element=w350:dbl)
              n256 = Index Array(array=w354, index=w346) -> (element=w355:dbl)
              n257 = Less?(x=w350, y=w348) -> (x < y?=w349:bool)
              n258 = Less Or Equal To 0?(x=w355) -> (x <= 0?=w353:bool)
              n259 = And(x=w353, y=w349) -> (x .and. y?=w347:bool)
            }
            n260 = flat-sequence {
              tunnel: [w324] -> w248
              tunnel: [w323] -> _
              tunnel: w245 -> [w323]
              tunnel: w247 -> [w322]
              tunnel: w246 -> [w321]
              tunnel: w245 -> [w318]
              tunnel: w244 -> [w315]
              tunnel: w243 -> [w314]
              tunnel: "Lambda" -> [w313]
              tunnel: w248 -> [w327]
              tunnel: w242 -> [w326]
              frame #0 {
                w320 = 0.06802721088435375  # AFR --> Lambda
                n261 = Multiply(x=w320, y=w315) -> (x*y=w319:dbl[])
                n262 = Select(t=w319, s=w313, f=w315) -> (s? t:f=w316:dbl[])
                n263 = control-ref of="AFR,EGT-Graph"() -> (w317:refnum<vi>)
                n264 = control-ref of="Leistungs-Graph"() -> (w324:refnum<vi>)
                n265 = call "UpdateGraph (SubVI).vi"("x"=w318, "Y2"=w314, "Y1"=w316, "XYGraph (Eingang)"=w317) -> ()  [unwired: 8 in]
                n266 = call "UpdateGraph (SubVI).vi"("x"=w323, "Y2"=w322, "Y1"=w321, "XYGraph (Eingang)"=w324) -> ()  [unwired: 8 in]
              }
              frame #1 {
                w339 = 1  # 0 = Keine Autoskalierung 1 = Autoskalierung
                w325 = 0
                w328 = 1
                w335 = 0
                n267 = Multiply(x=1.8, y=w326) -> (x*y=w329:dbl)
                n268 = property on="Eigenschaftsknoten" class="XYGraph (strikt)"(reference=w327, "ActYScl"=w335, "YScale.ScaleFit"=w328, "XScale.ScaleFit"=w328, "ActYScl"=w328, "YScale.Maximum"=w329, "YScale.Minimum"=w335) -> (reference out=w331:refnum<vi>)  [unwired: 1 in, 1 out]
                n269 = property on="Eigenschaftsknoten" class="XYGraph (strikt)"(reference=w331, "ActYScl"=w335) -> (reference out=w334:refnum<vi>, "YScale.Maximum"=w332:dbl, "XScale.Minimum"=w337:dbl, "XScale.Maximum"=w338:dbl)  [unwired: 1 in, 1 out]
                n270 = Add(x=w332, y=3.0) -> (x+y=w336:dbl)
                n271 = property on="Eigenschaftsknoten" class="XYGraph (strikt)"(reference=w334, "ActYScl"=w335, "YScale.Maximum"=w336) -> ()  [unwired: 1 in, 2 out]
                n272 = property on="AFR,EGT-Graph" class="XYGraph (strikt)"("XScale.Minimum"=w337, "XScale.Maximum"=w338, "ActYScl"=w325, "YScale.ScaleFit"=w325, "ActYScl"=w339, "YScale.ScaleFit"=w339) -> ()  [unwired: 2 in, 2 out]
              }
            }
            n273 = local read "Übersetzung ermitteln aus"() -> (w235:T2)
            n274 = Increment(x=w285) -> (x+1=w251:i32)
            n275 = Array Subset "nWelle"(array=w264, index=w251) -> (w268:dbl[])  [unwired: 1 in]
            n276 = Array Subset "EGT"(array=w253, index=w251) -> (w243:dbl[])  [unwired: 1 in]
            n277 = Array Subset "AFR"(array=w254, index=w251) -> (w244:dbl[])  [unwired: 1 in]
            n278 = Array Max & Min "nWelle_max [1/min]"(array=w268) -> (max value=w270:dbl)  [unwired: 3 out]
            n279 = Array Subset "n"(array=w265, index=w251) -> (w283:dbl[])  [unwired: 1 in]
            n280 = Array Subset "M"(array=w266, index=w251) -> (w275:dbl[])  [unwired: 1 in]
            n281 = Array Max & Min "Mmax"(array=w275) -> (max value=w238:dbl, max index (indices)=w284:i32)  [unwired: 2 out]
            n282 = Array Max & Min "nmax [1/min]"(array=w283) -> (max value=w274:dbl)  [unwired: 3 out]
            n283 = Array Subset "P"(array=w267, index=w251) -> (w246:dbl[])  [unwired: 1 in]
            n284 = Index Array "n(Mmax)"(array=w283, index=w284) -> (element=w237:dbl)
            n285 = Array Max & Min "Pmax"(array=w246) -> (max value=w255:dbl, max index (indices)=w269:i32)  [unwired: 2 out]
            "Pmax" <- w255
            n286 = call "n2v (SubVI).vi"("Übersetzung ermitteln aus"=w235, "Array (Eingang)"=w283, "Rollenumfang [m]"=w276) -> ("Array (Ausgang)"=w245:dbl[], "Boolesch"=w278:bool)  [unwired: 7 in]
            n287 = Index Array "nWelle (Pmax)"(array=w268, index=w269) -> (element=w259:dbl)
            n288 = Index Array "n(Pmax)"(array=w283, index=w269) -> (element=w258:dbl)
            n289 = case shown="Standard" w235 {
              tunnel: [w342 w345] -> w247
              tunnel: w275 -> [w342 _]
              tunnel: w268 -> [_ w345]
              tunnel: w238 -> [w341 _]
              tunnel: [w341 w344] -> w242
              tunnel: w270 -> [_ w344]
              tunnel: [w340 w343] -> w239
              tunnel: w259 -> [_ w343]
              tunnel: w258 -> [w340 _]
              frame Default {
              }
              frame "Vario (km/h)" {
              }
            }
            "n(Pmax)" <- w239
            n290 = Divide(x=w274, y=w233) -> (x/y=w291:dbl)
            n291 = local read "Lufttemperatur [°C]"() -> (w272:dbl)
            n292 = local read "Luftdruck [mbar]"() -> (w273:dbl)
            n293 = local read "Strecke [m]"() -> (w256:dbl)
            n294 = Compound Arithmetic op=MULTIPLY "v(Pmax)"(w258, w276, w277) -> (w236:dbl)
            n295 = Compound Arithmetic op=MULTIPLY "vmax"(w291, w276, w277) -> (w234:dbl)
            n296 = Format Date/Time String(time format string (%c)="%x %H:%M") -> (date/time string=w257:string)  [unwired: 2 in]
            "Datum+Zeit" <- w257
            n297 = Format Into String(format string="%.1f PS bei %d 1/min   |   %.1f Nm bei %d 1/min   |   vmax %d km/h\\nDIN 70020 k =%.3f (%d \\B0C, %d mbar)   |   %.0f m\\n%s" ("Format-String"), w255, w258, w238, w237, w234, w271, w272, w273, w256, w257) -> (resulting string=w281:string)  [unwired: 2 in, 1 out]
            n298 = Format Into String(format string="%.1f PS bei %d km/h, %d 1/min   |   vmax %d km/h\\nDIN 70020 k =%.3f (%d \\B0C, %d mbar)   |   %.0f m\\n%s" ("Format-String"), w255, w236, w259, w234, w271, w272, w273, w256, w257) -> (resulting string=w279:string)  [unwired: 2 in, 1 out]
            n299 = property on="Pmax" class="Str"("Text.FontSize"=48) -> ()  [unwired: 2 in, 2 out]
            n300 = Format Into String(format string="%.1f PS" ("Format-String"), w255) -> (resulting string=→"Pmax" →"PS_gross":string)  [unwired: 2 in, 1 out]
            n301 = Select(t=w279, s=w278, f=w281) -> (s? t:f=→"Ergebnis":string)
            n302 = case shown="\"Vario (km/h)\"" w235 {
              tunnel: w239 -> [w302 w308]
              tunnel: w238 -> [w299 _]
              tunnel: w237 -> [w296 _]
              tunnel: w236 -> [_ w307]
              tunnel: w234 -> [_ w305]
              frame Default {
                n303 = Format Into String(format string="%.1f Nm" ("Format-String"), w299) -> (resulting string=→"M_gross":string)  [unwired: 2 in, 1 out]
                n304 = Format Into String(format string="\\n    %d 1/min" ("Format-String"), w296) -> (resulting string=→"nM_gross":string)  [unwired: 2 in, 1 out]
                n305 = Format Into String(format string="\\n  %d 1/min" ("Format-String"), w302) -> (resulting string=→"nPS_gross":string)  [unwired: 2 in, 1 out]
              }
              frame "Vario (km/h)" {
                n306 = Format Into String(format string="%d km/h" ("Format-String"), w305) -> (resulting string=w310:string)  [unwired: 2 in, 1 out]
                n307 = Format Into String(format string="  %d km/h \\n  %d 1/min" ("Format-String"), w307, w308) -> (resulting string=w309:string)  [unwired: 2 in, 1 out]
                n308 = property on="nPS_gross" class="Str"("Value"=w309) -> ()  [unwired: 2 in, 2 out]
                n309 = property on="M_gross" class="Str"("Value"=w310) -> ()  [unwired: 2 in, 2 out]
                n310 = property on="nM_gross" class="Str"("Value"="") -> ()  [unwired: 2 in, 2 out]
              }
            }
          }
        }
        n311 = flat-sequence {
          tunnel: w61 -> [w181]
          tunnel: w25 -> [w174]
          tunnel: w26 -> [w175]
          tunnel: w62 -> [w176]
          tunnel: w63 -> [w182]
          tunnel: [w182] -> w83
          tunnel: [w176] -> w82
          tunnel: [w175] -> w81
          tunnel: [w174] -> w80
          tunnel: [w181] -> w79
          tunnel: [w178] -> w50
          tunnel: w49 -> [w178]
          tunnel: [w177] -> w42
          tunnel: w41 -> [w177]
          tunnel: w21 -> [w172]
          tunnel: w20 -> [w173]
          tunnel: [w173] -> w19
          tunnel: [w172] -> w18
          tunnel: w83 -> [w227]
          tunnel: w82 -> [w226]
          tunnel: w81 -> [w225]
          tunnel: w80 -> [w224]
          tunnel: w79 -> [w223]
          tunnel: w50 -> [w209]
          tunnel: w42 -> [w207]
          tunnel: w19 -> [w189]
          tunnel: w18 -> [w188]
          frame #0 {
            w180 = FALSE ("Start [F1]")
            w171 = 0  # Aktivieren
            n312 = property on="Überschrift Leistungsdiagramm" class="Str"() -> ("Value"=→"Titel_gross":string)  [unwired: 2 in, 2 out]
            n313 = property on="Fahrzeugdaten" class="Str"() -> ("Value"=→"Fahrzeugdaten_gross":string)  [unwired: 2 in, 2 out]
            n314 = property on="Drucken" class="Bool. (strikt)"("DisabledEnum"=w171) -> ()  [unwired: 2 in, 2 out]
            n315 = property on="Übersetzung ermitteln aus" class="Enum (strikt)"("DisabledEnum"=w171) -> ()  [unwired: 2 in, 2 out]
            n316 = property on="Grossbild schließen" class="Bool."("DisabledEnum"=w171) -> ()  [unwired: 2 in, 2 out]
            n317 = property on="Speichern" class="Bool. (strikt)"("DisabledEnum"=w171) -> ()  [unwired: 2 in, 2 out]
            n318 = property on="Konfiguration:" class="Bool. (strikt)"("DisabledEnum"=w171) -> ()  [unwired: 2 in, 2 out]
            n319 = property on="Ende" class="Bool. (strikt)"("DisabledEnum"=w171) -> ()  [unwired: 2 in, 2 out]
            n320 = property on="Titel_gross" class="Str"("Visible"="Grossbild") -> ()  [unwired: 2 in, 2 out]
            n321 = property on="Fahrzeugdaten_gross" class="Str"("Visible"="Grossbild") -> ()  [unwired: 2 in, 2 out]
            n322 = property on="(c)_gross" class="Str"("Visible"="Grossbild") -> ()  [unwired: 2 in, 2 out]
            n323 = property on="PS_gross" class="Str"("Visible"="Grossbild") -> ()  [unwired: 2 in, 2 out]
            n324 = property on="nPS_gross" class="Str"("Visible"="Grossbild") -> ()  [unwired: 2 in, 2 out]
            n325 = local write "Start"(w180) -> ()
            n326 = property on="Untersetzung\nermittelt" class="Bool. (strikt)"("BoolText.Text"="GO" ("Boolescher Text.Text"), "Blinking"=w180) -> ()  [unwired: 2 in, 2 out]
            n327 = local write "Untersetzung\nermittelt"(w180) -> ()
            n328 = property on="Grossbild schließen" class="Bool."("Visible"="Grossbild") -> ()  [unwired: 2 in, 2 out]
            n329 = property on="nM_gross" class="Str"("Visible"="Grossbild") -> ()  [unwired: 2 in, 2 out]
            n330 = property on="M_gross" class="Str"("Visible"="Grossbild") -> ()  [unwired: 2 in, 2 out]
          }
          frame #1 {
            # "Es können evtl. aus Datenspeicher noch Werte entfernt und für anderes verwendet werden,\nda einige in diesem VI nicht beschrieben und evlt. auch in ReCalc nicht verwendet werden\n(Ggf. auch in ReCalc prüfen ob das auch tatsächlich so ist!)"
            n331 = local read "Überschrift Leistungsdiagramm"() -> (w195:string)
            n332 = local read "Datum+Zeit"() -> (w199:string)
            n333 = local read "Lufttemperatur [°C]"() -> (w215:dbl)
            n334 = local read "Luftdruck [mbar]"() -> (w214:dbl)
            n335 = local read "Gleitender Mittelwert"() -> (w217:u8)
            n336 = local read "Differenzenquotient"() -> (w216:u8)
            n337 = local read "Übersetzung ermitteln aus"() -> (w184:T2)
            n338 = local read "Verlustmoment M1 [Nm] bei n1"() -> (w204:dbl)
            n339 = local read "Verlustmoment M0 [Nm] bei n = 0"() -> (w205:dbl)
            n340 = local read "Grossbild"() -> (w187:bool)
            n341 = Path To String(path="Auto-Pfad") -> (string=w202:string)
            n342 = local read "nKuWe/nRolle"() -> (w183:dbl)
            n343 = local read "Rollenträgheit [kgm²]"() -> (w221:dbl)
            n344 = local read "Rollendrehzahl n1 [1/min]"() -> (w206:u16)
            n345 = local read "Messung Klimadaten"() -> (w211:bool)
            n346 = local read "Reifenumfang [m]"() -> (w218:dbl)
            n347 = local read "n vom Gas [1/min]"() -> (w212:u16)
            n348 = local read "Zündung [Imp/U]"() -> (w220:dbl)
            n349 = local read "v vom Gas [km/h]"() -> (w208:u16)
            n350 = local read "AFR, EGT"() -> (w193:bool)
            n351 = local read "Getriebe [1:]"() -> (w219:dbl)
            n352 = Concatenate Strings(w199, "|", w202) -> (w201:string)
            n353 = local read "Lambda"() -> (w192:bool)
            n354 = local read "Dauer [s]"() -> (w213:u8)
            n355 = Boolean To (0,1)(Boolean=w187) -> (0, 1=w186:i16)
            n356 = local read "Rollengeber [Inkr/U]"() -> (w222:u16)
            n357 = To Double Precision Float(number=w186) -> (double precision float=w185:dbl)
            n358 = Build Array(w193, w192) -> (w191:bool[])
            n359 = local read "Strecke [m]"() -> (w198:dbl)
            n360 = Boolean Array To Number(Boolean array=w191) -> (number=w190:u32)
            n361 = Concatenate Strings("Fahrzeugdaten", "§$", w195) -> (w197:string)
            n362 = Bundle(w197, w201, "Rollengeber [Inkr/U]"=w222, "Rollenumfang [m]"=w225, "Rollenträgheit [kgm²]"=w221, "Zündung [Imp/U]"=w220, "Getriebe [1:]"=w219, "Reifenumfang [m]"=w218, w185, "Gleitender Mittelwert"=w217, "Differenzenquotient"=w216, w190, w227, "Strecke [m]"=w198, "Lufttemperatur [°C]"=w215, "Rollendrehzahl n1 [1/min]"=w206, "Luftdruck [mbar]"=w214, w226, w207, w189, w188, "Übersetzung ermitteln aus"=w184, "Dauer [s]"=w213, "Verlustmoment M0 [Nm] bei n = 0"=w205, "Verlustmoment M1 [Nm] bei n1"=w204, "n vom Gas [1/min]"=w212, w224, w223, "Messung Klimadaten"=w211, "VISA-Referenz (Ausgang)"=w209, "nKuWe/nRolle"=w183, "v vom Gas [km/h]"=w208) -> (→"Datenspeicher":T5)  [unwired: 1 in]
          }
          frame #2 {
            n363 = local read "Auto-Speichern"() -> (w230:bool)
            n364 = local read "Lauf abgebrochen"() -> (w229:bool)
            n365 = Not(x=w229) -> (.not. x?=w228:bool)
            n366 = And(x=w230, y=w228) -> (x .and. y?=w231:bool)
            n367 = case shown="True" w231 {
              frame False {
              }
              frame True {
                n368 = property on="Speichern" class="Bool. (strikt)"("Val(Sgnl)"=TRUE) -> ()  [unwired: 2 in, 2 out]
              }
            }
          }
        }
      }
    }
    n369 = local read "Ende"() -> (w14:bool)
  }
  n370 = flat-sequence {
    frame #0 {
      n371 = local read "Datenspeicher"() -> (w832:T3)
      n372 = call <vilib>:"Application Directory.vi"() -> ("Application Directory"=w853:path)
      n373 = Build Path(base path=w853, name or relative path="Konfig.xml") -> (appended path=w834:path)
      n374 = call "LoadCluster(SubVI)2.0.5.vi"("Datenspeicher"=w832, "XML File Path"=w834) -> ("Value"=w833:T3)  [unwired: 7 in, 2 out]
      n375 = property on="Datenspeicher" class="Cluster (strikt)"("Value"=w833) -> ()  [unwired: 2 in, 2 out]
      n376 = Unbundle(w833) -> ("Fahrzeugdaten"=w817:string, "Auto-Pfad"=w825:string, "Rolle [Inkr/U]"=w851:u16, "Rollenumfang [m]"=w850:dbl, "Rollenträgheit [kgm²]"=w849:dbl, "Zündung [Imp/U]"=w848:dbl, "Getriebe [1:]"=w847:dbl, "Reifenumfang [m]"=w846:dbl, "Grossanzeige"=w806:dbl, "Gl. Mittelwert"=w845:u8, "Differenzenquotient"=w844:u8, "AFR,EGT"=w810:u8, "Lufttemperatur [°C]"=w843:dbl, "Mv: n1 [1/min]"=w828:dbl, "Luftdruck [mbar]"=w842:dbl, "Übersetzung ermitteln aus"=w839:u8, "[s]"=w841:dbl, "Mv: M0 [Nm]"=w830:dbl, "Mv: M1 [Nm]"=w831:dbl, "n vom Gas [1/min]"=w840:dbl, "Boolesch"=w838:bool, "Serielle Schnittstelle"=w837:refnum<visa-resource-name>, "nKuWe/nRolle"=w836:dbl, "v vom Gas [km/h]"=w835:dbl)  [unwired: 8 out]
      n377 = property on="Dauer [s]" class="DigWert (strikt)"("Value"=w841) -> ()  [unwired: 2 in, 2 out]
      n378 = Not Equal To 0?(x=w806) -> (x != 0?=w807:bool)
      n379 = property on="Rollengeber [Inkr/U]" class="DigWert (strikt)"("Value"=w851) -> ()  [unwired: 2 in, 2 out]
      n380 = property on="Rollenumfang [m]" class="DigWert (strikt)"("Value"=w850) -> ()  [unwired: 2 in, 2 out]
      n381 = property on="Rollenträgheit [kgm²]" class="DigWert (strikt)"("Value"=w849) -> ()  [unwired: 2 in, 2 out]
      n382 = property on="Zündung [Imp/U]" class="DigWert (strikt)"("Value"=w848) -> ()  [unwired: 2 in, 2 out]
      n383 = property on="Getriebe [1:]" class="DigWert (strikt)"("Value"=w847) -> ()  [unwired: 2 in, 2 out]
      n384 = property on="Reifenumfang [m]" class="DigWert (strikt)"("Value"=w846) -> ()  [unwired: 2 in, 2 out]
      n385 = property on="Gleitender Mittelwert" class="DigWert (strikt)"("Value"=w845) -> ()  [unwired: 2 in, 2 out]
      n386 = property on="Differenzenquotient" class="DigWert (strikt)"("Value"=w844) -> ()  [unwired: 2 in, 2 out]
      n387 = property on="Lufttemperatur [°C]" class="DigWert (strikt)"("Value"=w843) -> ()  [unwired: 2 in, 2 out]
      n388 = property on="Luftdruck [mbar]" class="DigWert (strikt)"("Value"=w842) -> ()  [unwired: 2 in, 2 out]
      n389 = property on="Übersetzung ermitteln aus" class="Enum (strikt)"("Val(Sgnl)"=w839) -> ()  [unwired: 2 in, 2 out]
      n390 = property on="n vom Gas [1/min]" class="DigWert (strikt)"("Value"=w840) -> ()  [unwired: 2 in, 2 out]
      n391 = property on="Messung Klimadaten" class="Bool. (strikt)"("Val(Sgnl)"=w838) -> ()  [unwired: 2 in, 2 out]
      n392 = local write "Serielle Schnittstelle"(w837) -> ()
      n393 = property on="nKuWe/nRolle" class="DigWert (strikt)"("Value"=w836) -> ()  [unwired: 2 in, 2 out]
      n394 = property on="v vom Gas [km/h]" class="DigWert (strikt)"("Value"=w835) -> ()  [unwired: 2 in, 2 out]
      n395 = property on="Grossbild" class="Bool. (strikt)"("Value"=w807) -> ()  [unwired: 2 in, 2 out]
      n396 = Number To Boolean Array(number=w810) -> (Boolean array=w813:bool[])
      n397 = property on="Verlustmoment M0 [Nm] bei n = 0" class="DigWert (strikt)"("Value"=w830) -> ()  [unwired: 2 in, 2 out]
      n398 = property on="Verlustmoment M1 [Nm] bei n1" class="DigWert (strikt)"("Value"=w831) -> ()  [unwired: 2 in, 2 out]
      n399 = Index Array(array=w813, index=0) -> (element=w808:bool)
      n400 = Index Array(array=w813, index=1) -> (element=w809:bool)
      n401 = property on="AFR, EGT" class="Bool. (strikt)"("Val(Sgnl)"=w808) -> ()  [unwired: 2 in, 2 out]
      n402 = property on="Lambda" class="Bool. (strikt)"("Val(Sgnl)"=w809) -> ()  [unwired: 2 in, 2 out]
      n403 = Max & Min(x=1, y=w828) -> (max(x,y)=w827:dbl)  [unwired: 1 out]
      n404 = Search/Split String "führendes Datum+Zeit wegschneiden"(string=w825, search string/char (-)="|") -> (substring before match=w820:string, match + rest of string=w823:string)  [unwired: 1 in, 1 out]
      n405 = Search/Split String "führende Fahrzeugdaten wegschneiden"(string=w817, search string/char (-)="§$") -> (substring before match=w815:string, match + rest of string=w816:string)  [unwired: 1 in, 1 out]
      n406 = property on="Rollendrehzahl n1 [1/min]" class="DigWert (strikt)"("Value"=w827) -> ()  [unwired: 2 in, 2 out]
      n407 = String Subset(string=w823, offset (0)=1) -> (substring=w821:string)  [unwired: 1 in]
      n408 = String Subset(string=w816, offset (0)=2) -> (substring=w814:string)  [unwired: 1 in]
      n409 = String To Path(string=w821) -> (path=w826:path)
      n410 = property on="Fahrzeugdaten" class="Str"("Value"=w815) -> ()  [unwired: 2 in, 2 out]
      n411 = property on="Überschrift Leistungsdiagramm" class="Str"("Value"=w814) -> ()  [unwired: 2 in, 2 out]
      n412 = property on="Auto-Pfad" class="Pfad"("Value"=w826) -> ()  [unwired: 2 in, 2 out]
      n413 = property on="Datum+Zeit" class="Str"("Value"=w820) -> ()  [unwired: 2 in, 2 out]
    }
    frame #1 {
      w860 = 2  # Deaktivieren
      w862 = 0.0  # Graphen löschen
      n414 = local read "Serielle Schnittstelle"() -> (w858:refnum<visa-resource-name>)
      n415 = property on="Füllstand Lesepuffer" class="Schieber (strikt)"("Scale.Maximum"=100) -> ()  [unwired: 2 in, 2 out]
      n416 = property on="Frontpanel-Position" class="Bereich"("Origin"=T6 {"Horizontal"=8, "Vertical"=6}) -> ()  [unwired: 2 in, 2 out]
      n417 = property on="Drucken" class="Bool. (strikt)"("DisabledEnum"=w860) -> ()  [unwired: 2 in, 2 out]
      n418 = property on="Speichern" class="Bool. (strikt)"("DisabledEnum"=w860) -> ()  [unwired: 2 in, 2 out]
      n419 = Build Array(w862) -> (w861:dbl[])
      n420 = VISA Clear(VISA resource name=w858) -> (VISA resource name out=w857:refnum<visa-resource-name>, error out=w856:errorcluster)  [unwired: 1 in]
      n421 = property on="Untersetzung-Graph" class="SVDiagr (strikt)"("History Data"=w861) -> ()  [unwired: 2 in, 2 out]
      n422 = VISA Close(VISA resource name=w857, error in (no error)=w856) -> (error out=w855:errorcluster)
      n423 = case shown="Kein Fehler" w855 {
        tunnel: [T4."Enabled" ("Deaktiviert") T4."Disabled and Grayed Out" ("Deaktiviert")] -> w854
        frame No Error {
        }
        frame Error {
        }
      }
      n424 = property on="Start" class="Bool. (strikt)"("DisabledEnum"=w854) -> ()  [unwired: 2 in, 2 out]
    }
  }
  n425 = while {
    stop <- w871 stop-if-true
    n426 = Wait (ms)(milliseconds to wait=10) -> ()  [unwired: 1 out]
    n427 = local read "Übersetzung ermitteln aus"() -> (w869:T2)
    n428 = local read "Leistung"() -> (w870:bool)
    n429 = case shown="Standard" w869 {
      tunnel: [FALSE TRUE] -> w868
      frame Default {
      }
      frame "Vario (km/h)" {
      }
    }
    n430 = case shown="False" w870 {
      tunnel: w868 -> [w883 _]
      frame False {
        n431 = control-ref of="[°C]"() -> (w880:refnum<vi>)
        n432 = control-ref of="AFR"() -> (w881:refnum<vi>)
        n433 = control-ref of="Welle\n[1/min]"() -> (w887:refnum<vi>)
        n434 = control-ref of="Hinterrad\n[km/h]"() -> (w886:refnum<vi>)
        n435 = control-ref of="Ende"() -> (w885:refnum<vi>)
        n436 = control-ref of="Leistung"() -> (w884:refnum<vi>)
        n437 = control-ref of="Lambda"() -> (w879:refnum<vi>)
        n438 = control-ref of="AFR, EGT"() -> (w882:refnum<vi>)
        n439 = call "Tachomodus (SubVI).vi"("Lambda"=w879, "EGT"=w880, "AFR EGT"=w882, "AFR"=w881, "cvt"=w883, "Leistung"=w884, "Stopp"=w885, "Hinterrad"=w886, "Welle"=w887) -> ()  [unwired: 3 in]
      }
      frame True {
      }
    }
    n440 = case shown="True" "Rollendrehzahl aufzeichnen" {
      frame False {
      }
      frame True {
        n441 = control-ref of="Rollendrehzahl aufzeichnen"() -> (w875:refnum<vi>)
        n442 = control-ref of="Ende"() -> (w874:refnum<vi>)
        n443 = control-ref of="Cyclecounter"() -> (w873:refnum<vi>)
        n444 = control-ref of="dT"() -> (w872:refnum<vi>)
        n445 = control-ref of="n(Rolle) [1/min]"() -> (w876:refnum<vi>)
        n446 = call "Rollendrehzahl (SubVI).vi"("dT(Rolle) (Eingang)"=w872, "Cyclecounter"=w873, "Stop"=w874, "Rollendrehzahl aufzeichnen"=w875, "n(Rolle) (Eingang)"=w876) -> ()  [unwired: 7 in]
      }
    }
    n447 = local read "Ende"() -> (w871:bool)
  }
  n448 = property on="PS_gross" class="Str"("Visible"=w1) -> ()  [unwired: 2 in, 2 out]
  n449 = property on="Titel_gross" class="Str"("Visible"=w1) -> ()  [unwired: 2 in, 2 out]
  n450 = property on="Grossbild schließen" class="Bool."("Visible"=w1) -> ()  [unwired: 2 in, 2 out]
  n451 = property on="nPS_gross" class="Str"("Visible"=w1) -> ()  [unwired: 2 in, 2 out]
  n452 = property on="Fahrzeugdaten_gross" class="Str"("Visible"=w1) -> ()  [unwired: 2 in, 2 out]
  n453 = property on="nM_gross" class="Str"("Visible"=w1) -> ()  [unwired: 2 in, 2 out]
  n454 = property on="M_gross" class="Str"("Visible"=w1) -> ()  [unwired: 2 in, 2 out]
  n455 = property on="(c)_gross" class="Str"("Visible"=w1) -> ()  [unwired: 2 in, 2 out]
  n456 = property on="Auto-Speichern" class="Bool. (strikt)"("Value"=w4) -> ()  [unwired: 2 in, 2 out]
  n457 = property on="FahrzeugdatenZeichenzahl" class="DigWert (strikt)"("DisabledEnum"=T4."Disabled and Grayed Out" ("Deaktiviert")) -> ()  [unwired: 2 in, 2 out]
  n458 = while {
    stop <- w891 stop-if-true
    n459 = event shown="[7] \"Recalc\": Wertänderung" {
      selector: _ -> [_ _ _ _ _ _ _ _ _ _ _ _ _ _ _]
      dyn-events: _ -> [_ _ _ _ _ _ _ _ _ _ _ _ _ _ _]
      timeout: _ -> [_ _ _ _ _ _ _ _ _ _ _ _ _ _ _]
      tunnel: [_ _ _ TRUE _ _ _ _ _ _ _ _ _ _ _] -> w891
      event "Konfiguration:": Value Change {
        n460 = event-data() -> ("OldVal"=w893:bool)  [unwired: 1 in, 5 out]
        n461 = flat-sequence {
          tunnel: [w939] -> w894
          tunnel: w893 -> [w939]
          tunnel: w894 -> [w940]
          frame #0 {
            n462 = property on="Datenspeicher" class="Cluster (strikt)"() -> ("Value"=w938:T3)  [unwired: 2 in, 2 out]
            n463 = call "LoadCluster(SubVI)2.0.5.vi"("Datenspeicher"=w938) -> ("Value"=w937:T3)  [unwired: 8 in, 2 out]
            n464 = Unbundle(w937) -> ("Fahrzeugdaten"=w904:string, "Auto-Pfad"=w912:string, "Rolle [Inkr/U]"=w936:u16, "Rollenumfang [m]"=w935:dbl, "Rollenträgheit [kgm²]"=w934:dbl, "Zündung [Imp/U]"=w933:dbl, "Getriebe [1:]"=w932:dbl, "Reifenumfang [m]"=w931:dbl, "Grossanzeige"=w896:dbl, "Gl. Mittelwert"=w930:u8, "Differenzenquotient"=w929:u8, "AFR,EGT"=w897:u8, "Lufttemperatur [°C]"=w928:dbl, "Mv: n1 [1/min]"=w909:dbl, "Luftdruck [mbar]"=w927:dbl, "Übersetzung ermitteln aus"=w924:u8, "[s]"=w926:dbl, "Mv: M0 [Nm]"=w920:dbl, "Mv: M1 [Nm]"=w919:dbl, "n vom Gas [1/min]"=w925:dbl, "Boolesch"=w923:bool, "nKuWe/nRolle"=w922:dbl, "v vom Gas [km/h]"=w921:dbl)  [unwired: 9 out]
            n465 = property on="Dauer [s]" class="DigWert (strikt)"("Value"=w926) -> ()  [unwired: 2 in, 2 out]
            n466 = property on="Gleitender Mittelwert" class="DigWert (strikt)"("Value"=w930) -> ()  [unwired: 2 in, 2 out]
            n467 = property on="Übersetzung ermitteln aus" class="Enum (strikt)"("Val(Sgnl)"=w924) -> ()  [unwired: 2 in, 2 out]
            n468 = property on="Rollengeber [Inkr/U]" class="DigWert (strikt)"("Value"=w936) -> ()  [unwired: 2 in, 2 out]
            n469 = property on="Rollenumfang [m]" class="DigWert (strikt)"("Value"=w935) -> ()  [unwired: 2 in, 2 out]
            n470 = property on="Rollenträgheit [kgm²]" class="DigWert (strikt)"("Value"=w934) -> ()  [unwired: 2 in, 2 out]
            n471 = property on="Zündung [Imp/U]" class="DigWert (strikt)"("Value"=w933) -> ()  [unwired: 2 in, 2 out]
            n472 = property on="Getriebe [1:]" class="DigWert (strikt)"("Value"=w932) -> ()  [unwired: 2 in, 2 out]
            n473 = property on="Reifenumfang [m]" class="DigWert (strikt)"("Value"=w931) -> ()  [unwired: 2 in, 2 out]
            n474 = property on="Lufttemperatur [°C]" class="DigWert (strikt)"("Value"=w928) -> ()  [unwired: 2 in, 2 out]
            n475 = property on="Luftdruck [mbar]" class="DigWert (strikt)"("Value"=w927) -> ()  [unwired: 2 in, 2 out]
            n476 = property on="n vom Gas [1/min]" class="DigWert (strikt)"("Value"=w925) -> ()  [unwired: 2 in, 2 out]
            n477 = property on="Messung Klimadaten" class="Bool. (strikt)"("Val(Sgnl)"=w923) -> ()  [unwired: 2 in, 2 out]
            n478 = property on="nKuWe/nRolle" class="DigWert (strikt)"("Value"=w922) -> ()  [unwired: 2 in, 2 out]
            n479 = property on="v vom Gas [km/h]" class="DigWert (strikt)"("Value"=w921) -> ()  [unwired: 2 in, 2 out]
            n480 = property on="Differenzenquotient" class="DigWert (strikt)"("Value"=w929) -> ()  [unwired: 2 in, 2 out]
            n481 = Not Equal To 0?(x=w896) -> (x != 0?=w895:bool)
            n482 = Number To Boolean Array(number=w897) -> (Boolean array=w902:bool[])
            n483 = property on="Verlustmoment M1 [Nm] bei n1" class="DigWert (strikt)"("Value"=w919) -> ()  [unwired: 2 in, 2 out]
            n484 = property on="Verlustmoment M0 [Nm] bei n = 0" class="DigWert (strikt)"("Value"=w920) -> ()  [unwired: 2 in, 2 out]
            n485 = property on="Grossbild" class="Bool. (strikt)"("Value"=w895) -> ()  [unwired: 2 in, 2 out]
            n486 = Index Array(array=w902, index=0) -> (element=w899:bool)
            n487 = Index Array(array=w902, index=1) -> (element=w898:bool)
            n488 = property on="Lambda" class="Bool. (strikt)"("Val(Sgnl)"=w898) -> ()  [unwired: 2 in, 2 out]
            n489 = property on="AFR, EGT" class="Bool. (strikt)"("Value"=w899) -> ()  [unwired: 2 in, 2 out]
            n490 = Search/Split String "führende Fahrzeugdaten wegschneiden"(string=w904, search string/char (-)="§$") -> (substring before match=w903:string, match + rest of string=w906:string)  [unwired: 1 in, 1 out]
            n491 = Search/Split String "führendes Datum+Zeit wegschneiden"(string=w912, search string/char (-)="|") -> (substring before match=w913:string, match + rest of string=w916:string)  [unwired: 1 in, 1 out]
            n492 = Max & Min(x=1, y=w909) -> (max(x,y)=w911:dbl)  [unwired: 1 out]
            n493 = String Subset(string=w906, offset (0)=2) -> (substring=w905:string)  [unwired: 1 in]
            n494 = String Subset(string=w916, offset (0)=1) -> (substring=w914:string)  [unwired: 1 in]
            n495 = String To Path(string=w914) -> (path=w918:path)
            n496 = property on="Rollendrehzahl n1 [1/min]" class="DigWert (strikt)"("Value"=w911) -> ()  [unwired: 2 in, 2 out]
            n497 = property on="Überschrift Leistungsdiagramm" class="Str"("Value"=w905) -> ()  [unwired: 2 in, 2 out]
            n498 = property on="Datum+Zeit" class="Str"("Value"=w913) -> ()  [unwired: 2 in, 2 out]
            n499 = property on="Fahrzeugdaten" class="Str"("Value"=w903) -> ()  [unwired: 2 in, 2 out]
            n500 = property on="Auto-Pfad" class="Pfad"("Value"=w918) -> ()  [unwired: 2 in, 2 out]
          }
          frame #1 {
            n501 = property on="Konfiguration:" class="Bool. (strikt)"("Value"=w940) -> ()  [unwired: 2 in, 2 out]
          }
        }
      }
      event "Drucken": Value Change {
        n502 = event-data() -> ("OldVal"=w941:bool)  [unwired: 1 in, 5 out]
        n503 = flat-sequence {
          tunnel: [w949] -> w942
          tunnel: w941 -> [w949]
          tunnel: w942 -> [w950]
          frame #0 {
            n504 = control-ref of="Fahrzeugdaten"() -> (w947:refnum<vi>)
            n505 = control-ref of="Ergebnis"() -> (w946:refnum<vi>)
            n506 = control-ref of="Überschrift Leistungsdiagramm"() -> (w945:refnum<vi>)
            n507 = control-ref of="Leistungs-Graph"() -> (w948:refnum<vi>)
            n508 = control-ref of="AFR,EGT-Graph"() -> (w944:refnum<vi>)
            n509 = control-ref of="AFR, EGT"() -> (w943:refnum<vi>)
            n510 = call "printgraph_V0.01.vi"("AFR"=w943, "AFR-Graph (Eingang)"=w944, "Überschrift"=w945, "Ergebnis"=w946, "Fahrzeugdaten"=w947, "PM-Graph (Eingang)"=w948) -> ()  [unwired: 6 in]
          }
          frame #1 {
            n511 = property on="Drucken" class="Bool. (strikt)"("Value"=w950) -> ()  [unwired: 2 in, 2 out]
          }
        }
      }
      event "Speichern": Value Change {
        n512 = event-data() -> ("OldVal"=w951:bool)  [unwired: 1 in, 5 out]
        n513 = flat-sequence {
          frame #0 {
            n514 = property on="Auto-Gespeichert" class="Bool. (strikt)"("Value"=FALSE) -> ()  [unwired: 2 in, 2 out]
            n515 = property on="Auto-Datei" class="Str"("Value"="") -> ()  [unwired: 2 in, 2 out]
          }
          frame #1 {
            n516 = local read "Auto-Pfad"() -> (w965:path)
            n517 = property on="Auto-Speichern" class="Bool. (strikt)"() -> ("Value"=w960:bool)  [unwired: 2 in, 2 out]
            n518 = call <vilib>:"Check if File or Folder Exists.vi"("path"=w965) -> ("file or folder exists?"=w964:bool, "dup path"=w961:path)  [unwired: 8 in, 1 out]
            n519 = Not(x=w964) -> (.not. x?=w963:bool)
            n520 = And(x=w960, y=w963) -> (x .and. y?=w962:bool)
            n521 = And(x=w960, y=w964) -> (x .and. y?=w957:bool)
            n522 = case shown="True" w957 {
              tunnel: [path "" w988] -> w956
              tunnel: w961 -> [_ w987]
              tunnel: ["" w971] -> w958
              frame False {
              }
              frame True {
                n523 = local read "FahrzeugdatenZeichenzahl"() -> (w979:u8)
                n524 = local read "Fahrzeugdaten"() -> (w978:string)
                n525 = Get Date/Time In Seconds() -> (seconds since 1Jan1904=w991:timestamp)
                n526 = local read "Pmax"() -> (w984:dbl)
                n527 = local read "n(Pmax)"() -> (w983:dbl)
                n528 = Path To String(path=w987) -> (string=w990:string)
                n529 = Pick Line "Erste Zeile"(multi-line string=w978, line index=0) -> (output string=w972:string)  [unwired: 1 in]
                n530 = Format Into String(format string="%,;%.1f_%d" ("Format-String"), w984, w983) -> (resulting string=w980:string)  [unwired: 2 in, 1 out]
                n531 = String Subset "Anzahl\nZeichen"(string=w972, length (rest)=w979) -> (substring=w974:string)  [unwired: 1 in]
                n532 = Format Date/Time String(time format string (%c)="%y%m%d_%H%M%S_", seconds (now)=w991) -> (date/time string=w981:string)  [unwired: 1 in]
                n533 = String Length(string=w974) -> (length=w970:i32)
                n534 = Greater Than 0?(x=w970) -> (x > 0?=w976:bool)
                n535 = case shown="True" w976 {
                  tunnel: ["" w995] -> w975
                  tunnel: w974 -> [_ w993]
                  frame False {
                  }
                  frame True {
                    n536 = Concatenate Strings("_", w993) -> (w995:string)
                  }
                }
                n537 = Concatenate Strings(w981, w980, w975, ".xml") -> (w971:string)
                n538 = Concatenate Strings(w990, "\\", w971) -> (w989:string)
                n539 = String To Path(string=w989) -> (path=w988:path)
              }
            }
            n540 = control-ref of="Datenspeicher"() -> (w954:refnum<vi>)
            n541 = call "SaveCluster.vi"("selected path"=w956, "Datenspeicher"=w954) -> ("Kein Fehler"=w955:bool)
            n542 = And(x=w957, y=w955) -> (x .and. y?=w959:bool)
            n543 = case shown="True" w959 {
              tunnel: w958 -> [_ w967]
              frame False {
              }
              frame True {
                n544 = property on="Auto-Gespeichert" class="Bool. (strikt)"("Value"=TRUE) -> ()  [unwired: 2 in, 2 out]
                n545 = property on="Auto-Datei" class="Str"("Value"=w967) -> ()  [unwired: 2 in, 2 out]
              }
            }
            n546 = call "Meldung an Benutzer2"("Enable"=w962) -> ()  [unwired: 9 in, 2 out]
          }
        }
        n547 = local write "Speichern"(w951) -> ()
      }
      event "Ende": Value Change {
        n548 = event-data() -> ("OldVal"=w1004:bool)  [unwired: 1 in, 5 out]
        n549 = local read "Datenspeicher"() -> (w1006:T3)
        n550 = flat-sequence {
          tunnel: w1004 -> [w1034]
          tunnel: [w1034] -> w1003
          frame #0 {
            n551 = Wait (ms)(milliseconds to wait=u32 200) -> ()  [unwired: 1 out]
          }
        }
        n552 = Unbundle By Name(w1006) -> ("Auto-Pfad"=w998:string, "Rolle [Inkr/U]"=w1026:u16, "Rollenumfang [m]"=w1025:dbl, "Rollenträgheit [kgm²]"=w1024:dbl, "Zündung [Imp/U]"=w1023:dbl, "Getriebe [1:]"=w1022:dbl, "Reifenumfang [m]"=w1021:dbl, "Grossanzeige"=w996:dbl, "Gl. Mittelwert"=w1020:u8, "Differenzenquotient"=w1019:u8, "Fahrzeugdaten"=w1018:string, "Lufttemperatur [°C]"=w1017:dbl, "Mv: n1 [1/min]"=w1016:dbl, "Luftdruck [mbar]"=w1014:dbl, "nRolle"=w1015:dbl[], "Übersetzung ermitteln aus"=w1013:u8, "[s]"=w1012:dbl, "Mv: M0 [Nm]"=w1011:dbl, "Mv: M1 [Nm]"=w1010:dbl, "n vom Gas [1/min]"=w1009:dbl, "Boolesch"=w1008:bool, "Serielle Schnittstelle"=w1005:refnum<visa-resource-name>, "nWelle"=w1002:dbl[], "AFR"=w1000:dbl[], "EGT"=w999:dbl[], "v vom Gas [km/h]"=w1001:dbl, "AFR,EGT"=w997:u8)
        n553 = local write "Ende"(w1003) -> ()
        n554 = Bundle By Name(cluster=w1006, "Auto-Pfad"=w998, "Rolle [Inkr/U]"=w1026, "Rollenumfang [m]"=w1025, "Rollenträgheit [kgm²]"=w1024, "Zündung [Imp/U]"=w1023, "Getriebe [1:]"=w1022, "Reifenumfang [m]"=w1021, "Grossanzeige"=w996, "Gl. Mittelwert"=w1020, "Differenzenquotient"=w1019, "Fahrzeugdaten"=w1018, "Lufttemperatur [°C]"=w1017, "Mv: n1 [1/min]"=w1016, "Luftdruck [mbar]"=w1014, "nRolle"=w1015, "Übersetzung ermitteln aus"=w1013, "[s]"=w1012, "Mv: M0 [Nm]"=w1011, "Mv: M1 [Nm]"=w1010, "n vom Gas [1/min]"=w1009, "Boolesch"=w1008, "Serielle Schnittstelle"=w1005, "nWelle"=w1002, "AFR"=w1000, "EGT"=w999, "v vom Gas [km/h]"=w1001, "AFR,EGT"=w997) -> (w1007:T3)
        n555 = call <vilib>:"Application Directory.vi"() -> ("Application Directory"=w1029:path)
        n556 = Build Path(base path=w1029, name or relative path="Konfig.xml") -> (appended path=w1027:path)
        n557 = Flatten To XML(anything=w1007) -> (xml string=w1031:string)
        n558 = call-poly <vilib>:"Write to XML File.vi"("XML Input"=w1031, "XML File Path"=w1027) -> ("error out"=w1030:errorcluster)  [unwired: 7 in, 2 out]
        n559 = case shown="Kein Fehler" w1030 {
          frame No Error {
          }
          frame Error {
          }
        }
      }
      event "Serielle Schnittstelle": Value Change {
        n560 = event-data() -> ()  [unwired: 1 in, 6 out]
        n561 = property on="Start" class="Bool. (strikt)"("DisabledEnum"=T4."Enabled" ("Deaktiviert")) -> ()  [unwired: 2 in, 2 out]
      }
      event "Messung Klimadaten": Value Change {
        n562 = event-data() -> ("NewVal"=w1036:bool)  [unwired: 1 in, 5 out]
        n563 = case shown="True" w1036 {
          frame True {
            w1037 = T4."Disabled and Grayed Out" ("Deaktiviert")
            n564 = property on="Lufttemperatur [°C]" class="DigWert (strikt)"("DisabledEnum"=w1037) -> ()  [unwired: 2 in, 2 out]
            n565 = property on="Luftdruck [mbar]" class="DigWert (strikt)"("DisabledEnum"=w1037) -> ()  [unwired: 2 in, 2 out]
          }
          frame False {
            w1038 = T4."Enabled" ("Deaktiviert")
            n566 = property on="Lufttemperatur [°C]" class="DigWert (strikt)"("DisabledEnum"=w1038) -> ()  [unwired: 2 in, 2 out]
            n567 = property on="Luftdruck [mbar]" class="DigWert (strikt)"("DisabledEnum"=w1038) -> ()  [unwired: 2 in, 2 out]
          }
        }
      }
      event "Spenden": Value Change {
        n568 = event-data() -> ()  [unwired: 1 in, 6 out]
        n569 = case shown="True" "Spenden" {
          frame False {
          }
          frame True {
            w1040 = "https://www.paypal.com/cgi-bin/webscr?cmd=_s-xclick&hosted_button_id=5HCL4L3EEXS64&source=url"  # GruA
            (unwired) "https://www.paypal.com/cgi-bin/webscr?cmd=_s-xclick&hosted_button_id=8SA7Y5J5P5N3W&source=url" ("URL")
            n570 = call-poly <vilib>:"Open URL in Default Browser.vi"("URL"=w1040) -> ()  [unwired: 5 in, 2 out]
          }
        }
      }
      event "Recalc": Value Change {
        n571 = event-data() -> ("OldVal"=w1043:bool)  [unwired: 1 in, 5 out]
        n572 = property on="Recalc" class="Bool. (strikt)"("Value"=w1043) -> ()  [unwired: 2 in, 2 out]
        n573 = property on="Datenspeicher" class="Cluster (strikt)"() -> ("Value"=w1041:T3)  [unwired: 2 in, 2 out]
        n574 = call "ReCalc_V2.00.vi"("Berechnen"=TRUE, "Datenspeicher"=w1041) -> ()  [unwired: 3 in]
      }
      event "Übersetzung ermitteln aus": Value Change {
        n575 = event-data() -> ("NewVal"=w1057:T2)  [unwired: 1 in, 5 out]
        n576 = case shown="\"Vario (km/h)\"" w1057 {
          tunnel: [w1073 w1074 w1076 w1079] -> w1058
          tunnel: [w1073 w1075 w1076 w1078] -> w1053
          tunnel: [w1073 w1074 w1077 w1078] -> w1044
          tunnel: [w1073 w1075 w1077 w1079] -> w1052
          tunnel: [T4."Enabled" ("Deaktiviert") w1074 w1076 w1078] -> w1051
          frame "Vario (km/h)" {
            w1073 = T4."Disabled and Grayed Out" ("Deaktiviert")
          }
          frame "nKuWe / nRolle" {
            w1075 = T4."Enabled" ("Deaktiviert")
            w1074 = T4."Disabled and Grayed Out" ("Deaktiviert")
          }
          frame "Zündsignal", Default {
            w1077 = T4."Enabled" ("Deaktiviert")
            w1076 = T4."Disabled and Grayed Out" ("Deaktiviert")
          }
          frame "Getriebe & Reifen" {
            w1078 = T4."Disabled and Grayed Out" ("Deaktiviert")
            w1079 = T4."Enabled" ("Deaktiviert")
          }
        }
        n577 = case shown="Standard" w1057 {
          tunnel: ["n [1/min]" "M [Nm]"] -> w1056
          tunnel: [200.0 14000.0] -> w1055
          tunnel: ["v [km/h]" "n [1/min]"] -> w1050
          tunnel: [14000.0 60.0] -> w1049
          tunnel: [u32 16777216 w1067] -> w1047
          tunnel: [u32 16711680 w1067] -> w1046
          tunnel: [FALSE TRUE] -> w1045
          frame "Vario (km/h)" {
          }
          frame Default {
            w1067 = u32 9868950
          }
        }
        n578 = property on="Text Zündung" class="Str"("Text.TextColor"=w1046) -> ()  [unwired: 2 in, 2 out]
        n579 = property on="Welle [1/min]" class="Drehknopf (strikt)"("Active Slider"=1, "FG Color"=w1047) -> ()  [unwired: 2 in, 2 out]
        n580 = property on="Text Rolle" class="Str"("Visible"=w1045) -> ()  [unwired: 2 in, 2 out]
        n581 = property on="Leistungs-Graph" class="XYGraph (strikt)"("ActYScl"=1, "YScale.NameLbl.Text"=w1056, "YScale.Maximum"=w1049, "XScale.NameLbl.Text"=w1050, "XScale.Maximum"=w1055) -> ()  [unwired: 2 in, 2 out]
        n582 = property on="nKuWe/nRolle" class="DigWert (strikt)"("DisabledEnum"=w1053) -> ()  [unwired: 2 in, 2 out]
        n583 = property on="v vom Gas [km/h]" class="DigWert (strikt)"("DisabledEnum"=w1051) -> ()  [unwired: 2 in, 2 out]
        n584 = property on="n vom Gas [1/min]" class="DigWert (strikt)"("DisabledEnum"=w1052) -> ()  [unwired: 2 in, 2 out]
        n585 = property on="Getriebe [1:]" class="DigWert (strikt)"("DisabledEnum"=w1058) -> ()  [unwired: 2 in, 2 out]
        n586 = property on="Reifenumfang [m]" class="DigWert (strikt)"("DisabledEnum"=w1058) -> ()  [unwired: 2 in, 2 out]
        n587 = property on="Zündung [Imp/U]" class="DigWert (strikt)"("DisabledEnum"=w1044) -> ()  [unwired: 2 in, 2 out]
        n588 = property on="Dauer [s]" class="DigWert (strikt)"("DisabledEnum"=w1044) -> ()  [unwired: 2 in, 2 out]
        n589 = property on="Filter Zündsignal" class="Bool. (strikt)"("DisabledEnum"=w1044) -> ()  [unwired: 2 in, 2 out]
      }
      event "Reset Skalierung": Value Change {
        w1083 = 1
        w1082 = 0.0
        n590 = event-data() -> ()  [unwired: 1 in, 6 out]
        n591 = local read "Übersetzung ermitteln aus"() -> (w1088:T2)
        n592 = local read "Lambda"() -> (w1080:bool)
        n593 = case shown="Standard" w1088 {
          tunnel: [14000.0 200.0] -> w1081
          tunnel: [60.0 14000.0] -> w1087
          frame Default {
          }
          frame "Vario (km/h)" {
          }
        }
        n594 = case shown="False" w1080 {
          tunnel: [20.0 1.6] -> w1085
          tunnel: [10.0 0.4] -> w1084
          frame False {
          }
          frame True {
          }
        }
        n595 = property on="Leistungs-Graph" class="XYGraph (strikt)"("XScale.Maximum"=w1081, "XScale.Minimum"=w1082, "ActYScl"=w1082, "YScale.Maximum"=30.0, "YScale.Minimum"=w1082, "ActYScl"=w1083, "YScale.Maximum"=w1087, "YScale.Minimum"=w1082) -> ()  [unwired: 2 in, 2 out]
        n596 = property on="AFR,EGT-Graph" class="XYGraph (strikt)"("XScale.Maximum"=w1081, "XScale.Minimum"=w1082, "ActYScl"=w1082, "YScale.Maximum"=w1085, "YScale.Minimum"=w1084, "ActYScl"=w1083, "YScale.Maximum"=800.0, "YScale.Minimum"=w1082) -> ()  [unwired: 2 in, 2 out]
      }
      event "Auto-Speichern": Value Change {
        n597 = event-data() -> ("NewVal"=w1099:bool)  [unwired: 1 in, 5 out]
        n598 = case shown="True" w1099 {
          tunnel: [T4."Disabled and Grayed Out" ("Deaktiviert") w1101] -> w1098
          frame False {
          }
          frame True {
            n599 = local read "Auto-Pfad"() -> (w1104:path)
            n600 = call <vilib>:"Check if File or Folder Exists.vi"("path"=w1104) -> ("file or folder exists?"=w1102:bool)  [unwired: 8 in, 2 out]
            n601 = Not(x=w1102) -> (.not. x?=w1103:bool)
            n602 = case shown="False" w1102 {
              tunnel: [T4."Disabled and Grayed Out" ("Deaktiviert") T4."Enabled" ("Deaktiviert")] -> w1101
              frame False {
              }
              frame True {
              }
            }
            n603 = call "Meldung an Benutzer"("Enable"=w1103) -> ()  [unwired: 9 in, 2 out]
            n604 = local write "Auto-Speichern"(w1102) -> ()
          }
        }
        n605 = property on="FahrzeugdatenZeichenzahl" class="DigWert (strikt)"("DisabledEnum"=w1098) -> ()  [unwired: 2 in, 2 out]
      }
      event "Fahrzeugdaten": Value Change {
        # "Fahrzeugdaten auf 3 Zeilen begrenzen\n(Recalc ist nur auf max. 3 Zeilen ausgelegt)"
        n606 = event-data() -> ("OldVal"=w1109:string, "NewVal"=w1110:string)  [unwired: 1 in, 4 out]
        n607 = Spreadsheet String To Array(delimiter (Tab)="\n", format string="%s", spreadsheet string=w1110, array type (2D Dbl)=string[] []) -> (array=w1112:string[])
        n608 = Array Size "Zeilenanzahl"(array=w1112) -> (size(s)=w1111:i32)
        n609 = Greater?(x=w1111, y=3) -> (0:w1108:bool)
        n610 = case shown="True" w1108 {
          tunnel: w1109 -> [_ w1116]
          frame False {
          }
          frame True {
            n611 = flat-sequence {
              tunnel: w1116 -> [w1118]
              frame #0 {
                n612 = call "Meldung an Benutzer3"("Enable"=TRUE) -> ()  [unwired: 9 in, 2 out]
              }
              frame #1 {
                n613 = property on="Fahrzeugdaten" class="Str"("Value"=w1118) -> ()  [unwired: 2 in, 2 out]
              }
            }
          }
        }
      }
      event "AFR, EGT": Value Change {
        n614 = event-data() -> ("NewVal"=w1127:bool)  [unwired: 1 in, 5 out]
        n615 = local read "Höhe Leistungs-Graph (646)"() -> (w1123:u32)
        n616 = local read "Y-Koord. Graph-Reset-Button (782)"() -> (w1124:i32)
        n617 = control-ref of="Leistungs-Graph"() -> (w1126:refnum<vi>)
        n618 = control-ref of="Reset Skalierung"() -> (w1125:refnum<vi>)
        n619 = control-ref of="AFR,EGT-Graph"() -> (w1122:refnum<vi>)
        n620 = control-ref of="AFR"() -> (w1120:refnum<vi>)
        n621 = control-ref of="[°C]"() -> (w1119:refnum<vi>)
        n622 = control-ref of="Lambda"() -> (w1128:refnum<vi>)
        n623 = call "Enable_AFR_EGT_Graph (SubVI).vi"("Leistungsgraph"=w1126, "AFR EGT"=w1127, "Y-Koord. Graph-Reset-Button (782)"=w1124, "Lambda"=w1128, "Reset Skalierung"=w1125, "Höhe Leistungs-Graph (646)"=w1123, "AFR EGT Gaph"=w1122, "AFR"=w1120, "EGT [°C]"=w1119, "Skalierungsfaktor Leistungsgraph"=0.6666666666666666) -> ()  [unwired: 6 in]
      }
      event "Lambda": Value Change {
        w1131 = 14.7
        w1137 = 0.06802721088435375
        w1148 = 0
        n624 = event-data() -> ("NewVal"=w1133:bool)  [unwired: 1 in, 5 out]
        n625 = case shown="False" w1133 {
          tunnel: ["AFR" "l"] -> w1160
          tunnel: ["Anwendung" "Symbol"] -> w1159
          tunnel: [w1167 1.6] -> w1158
          tunnel: [w1166 0.4] -> w1165
          tunnel: [1 2] -> w1157
          tunnel: [0 1] -> w1163
          tunnel: [w1167 1.5] -> w1162
          tunnel: [w1166 0.5] -> w1161
          frame False {
            w1166 = 10.0
            w1167 = 20.0
          }
          frame True {
          }
        }
        n626 = property on="AFR,EGT-Graph" class="XYGraph (strikt)"("ActYScl"=w1148, "YScale.NameLbl.Text"=w1160, "YScale.NameLbl.FontName"=w1159, "YScale.Maximum"=w1158, "YScale.Minimum"=w1165, "YScale.Precision"=w1157) -> ("Height"=w1151:u32, "YScale.NameLbl.Width"=w1150:u32, "Top"=w1149:i32)  [unwired: 2 in, 2 out]
        n627 = property on="AFR" class="Drehknopf (strikt)"("Caption.Text"=w1160, "Caption.FontName"=w1159, "Scale.Maximum"=w1162, "Scale.Minimum"=w1161, "Scale.Format"=0, "Scale.Precision"=w1163) -> ()  [unwired: 2 in, 2 out]
        n628 = property on="AFR Zahlenanzeige" class="DigWert (strikt)"("Precision"=w1157) -> ()  [unwired: 2 in, 2 out]
        n629 = local read "AFR,EGT-Graph"() -> (w1136:cluster{dbl[], dbl[]}[])
        n630 = Subtract(x=w1151, y=w1150) -> (x-y=w1156:u32)
        n631 = Divide(x=w1156, y=2) -> (x/y=w1154:dbl)
        n632 = Add(x=w1154, y=w1149) -> (x+y=w1153:dbl)
        n633 = Index Array(array=w1136, index=1) -> (element=w1138:cluster{dbl[], dbl[]})
        n634 = Index Array(array=w1136, index=0) -> (element=w1146:cluster{dbl[], dbl[]})
        n635 = property on="AFR,EGT-Graph" class="XYGraph (strikt)"("ActYScl"=w1148, "YScale.NameLbl.Top"=w1153, "Active Plot"=0) -> ()  [unwired: 2 in, 2 out]
        n636 = local read "AFR"() -> (w1130:dbl)
        n637 = Unbundle(w1146) -> (w1140:dbl[], w1143:dbl[])
        n638 = Multiply(x=w1137, y=w1130) -> (x*y=w1129:dbl)
        n639 = Multiply(x=w1130, y=w1131) -> (x*y=w1134:dbl)
        n640 = Multiply(x=w1137, y=w1143) -> (x*y=w1144:dbl[])
        n641 = Multiply(x=w1131, y=w1143) -> (x*y=w1142:dbl[])
        n642 = Select(t=w1144, s=w1133, f=w1142) -> (s? t:f=w1141:dbl[])
        n643 = Select(t=w1129, s=w1133, f=w1134) -> (s? t:f=w1132:dbl)
        n644 = Bundle(w1140, w1141) -> (w1139:cluster{dbl[], dbl[]})  [unwired: 1 in]
        n645 = local write "AFR"(w1132) -> ()
        n646 = Build Array(w1139, w1138) -> (w1135:cluster{dbl[], dbl[]}[])
        n647 = property on="AFR,EGT-Graph" class="XYGraph (strikt)"("Value"=w1135) -> ()  [unwired: 2 in, 2 out]
      }
      event "Grossbild schließen": Value Change {
        w1180 = FALSE
        n648 = event-data() -> ()  [unwired: 1 in, 6 out]
        n649 = property on="Grossbild schließen" class="Bool."("Visible"=w1180) -> ()  [unwired: 2 in, 2 out]
        n650 = property on="(c)_gross" class="Str"("Visible"=w1180) -> ()  [unwired: 2 in, 2 out]
        n651 = property on="Fahrzeugdaten_gross" class="Str"("Visible"=w1180) -> ()  [unwired: 2 in, 2 out]
        n652 = property on="nM_gross" class="Str"("Visible"=w1180) -> ()  [unwired: 2 in, 2 out]
        n653 = property on="Titel_gross" class="Str"("Visible"=w1180) -> ()  [unwired: 2 in, 2 out]
        n654 = property on="nPS_gross" class="Str"("Visible"=w1180) -> ()  [unwired: 2 in, 2 out]
        n655 = property on="M_gross" class="Str"("Visible"=w1180) -> ()  [unwired: 2 in, 2 out]
        n656 = property on="PS_gross" class="Str"("Visible"=w1180) -> ()  [unwired: 2 in, 2 out]
      }
    }
    n657 = property class="Anw"() -> ("App.Kind"=w889:T7)  [unwired: 2 in, 2 out]
    n658 = Greater?(x=w889, y=1) -> (0:w890:bool)
    n659 = case shown="True" w890 {
      tunnel: w891 -> [_ w892]
      frame False {
      }
      frame True {
        n660 = Quit LabVIEW(quit? (T)=w892) -> ()
      }
    }
  }
  "Text Zündung" <- "Zündung"
  "Text Rolle" <- "Rolle"
  "Auto-Gespeichert" <- w4
  "Auto-Datei" <- ""
